vi "4Pi Objective Lock - EMBL_v2.vi"(7 "Calling VI Ref":refnum<vi>) -> ()   [LabVIEW 2021]
uses:
  <vilib>/Utility/miscctls.llb/LVPointTypeDef.ctl
  4Pi Objective Lock Type Defs/4Pi Obj Lock - Notifier Type.ctl
  4Pi Objective Lock Type Defs/4Pi Obj Lock - Actions.ctl
  <vilib>/vision/Image Controls.llb/IMAQ Image.ctl
  4Pi Objective Lock Type Defs/4Pi Obj Lock - Lock Settings.ctl
  Hardware Configuration/Hardware Configuration Controls/Device Type.ctl
  Hardware Configuration/Hardware Configuration Controls/Device Function.ctl
  4Pi Objective Lock Type Defs/4Pi Obj Lock - Camera Settings.ctl
  Device Library/Cameras/Camera Controls/Generic Camera ROI.ctl
  Device Library/Cameras/Camera Controls/Generic Camera Actions.ctl
  Device Manager/Common Device Queue/Common Device Controls/Common Device Actions.ctl
  Device Library/Stages/Stages Controls/Stage Actions.ctl
  <vilib>/addons/control/pid/pid.llb/PID (DBL Array).vi
  <vilib>/addons/control/pid/pid.llb/PID (DBL).vi
  <vilib>/addons/control/pid/NI_PID_pid.lvlib
  <vilib>/vision/NI_Vision_Development_Module.lvlib
panel:
  out "dz (µm)":dbl format="%.2f"
  out "dxy (px)":dbl[](array[numeric])
  in  "Main Tab":T1(tab)
  out "CC Max":cluster{"pixel size (µm)":dbl}(graph)
  out "Z Move":bool
  out "XY Move":bool
  out "Measured X Position (px)":dbl=1.0 format="%.3g"
  out "Measured Y Position (px)":dbl=1.0 format="%.3g"
  out "Measured sx/sy":dbl=1.0 format="%.3g"
  out "Target X Position (px)":dbl=1.0 format="%.3g"
  out "Target Y Position (px)":dbl=1.0 format="%.3g"
  out "Target sx/sy":dbl=1.0 format="%.3g"
  out "Z Axis Position (µm)":dbl=1.0 format="%.4g"
  out "Y Axis Position (µm)":dbl=1.0 format="%.2g"
  out "X Axis Position (µm)":dbl=1.0 format="%.2g"
  out "Z Target and Fit Value (µm)":T2(graph)
  in  "Start Lock":bool
  out "Y Target and Fit Position (µm)":T2(graph)
  out "X Target and Fit Position (µm)":T2(graph)
  in  "Restart Lock":bool
  out "Fit Error":bool
  out "Move Limit Error":bool
  out "dt z (s)":dbl format="%.3f"
  in  "Metric scale sx/sy":dbl=0.4
  in  "pixel size (µm)":dbl=0.05
  in  "X Update Scale Factor":dbl=0.005
  in  "Y Update Scale Factor":dbl=0.007
  in  "Z Update Scale Factor":dbl=0.4
  in  "Sample Z Step No.":u32=2
  in  "Sample Z Step Size (µm)":dbl=2.0
  in  "Update Delay (ms)":i32=10
  in  "D (Derivative)":dbl
  in  "I (Integral)":dbl
  in  "P (Proportional)":dbl=2.0
  in  "Invert Z Axis":bool
  in  "XY Drift Threshold":dbl=0.05
  in  "Abort If Error":bool
  in  "Flip XY Axis":bool
  in  "Invert X Axis":bool=TRUE
  in  "Invert Y Axis":bool=TRUE
  in  "Z Stage Move Limit (µm)":dbl=5.0
  in  "Z Drift Threshold":dbl=0.05
  in  "XY Stage Move Limit (µm)":dbl=1.0
  in  "Frame Accumulations":u16=10
  in  "XY Correction Active":bool=TRUE
  in  "Z Correction Active":bool=TRUE
  in  "Set Camera ROI":bool
  in  "Save Lock Settings":bool
  in  "Camera Settings":bool
  out "Target Y Position cc (px)":dbl=1.0 format="%.3g"
  out "Measured Y Position cc (px)":dbl=1.0 format="%.3g"
  out "Measured X Position cc (px)":dbl=1.0 format="%.3g"
  out "Target X Position cc (px)":dbl=1.0 format="%.3g"
  out "Target Z (µm)":dbl=1.0 format="%.3g"
  out "Measured Z (µm)":dbl=1.0 format="%.3g"
  out "CC Max Value":dbl=1.0 format="%.3g"
  in  "Quit":bool
  # "Z Drift Settings"
  # "XY Drift Settings"
  # "PID Control Values"
  # "General Settings"
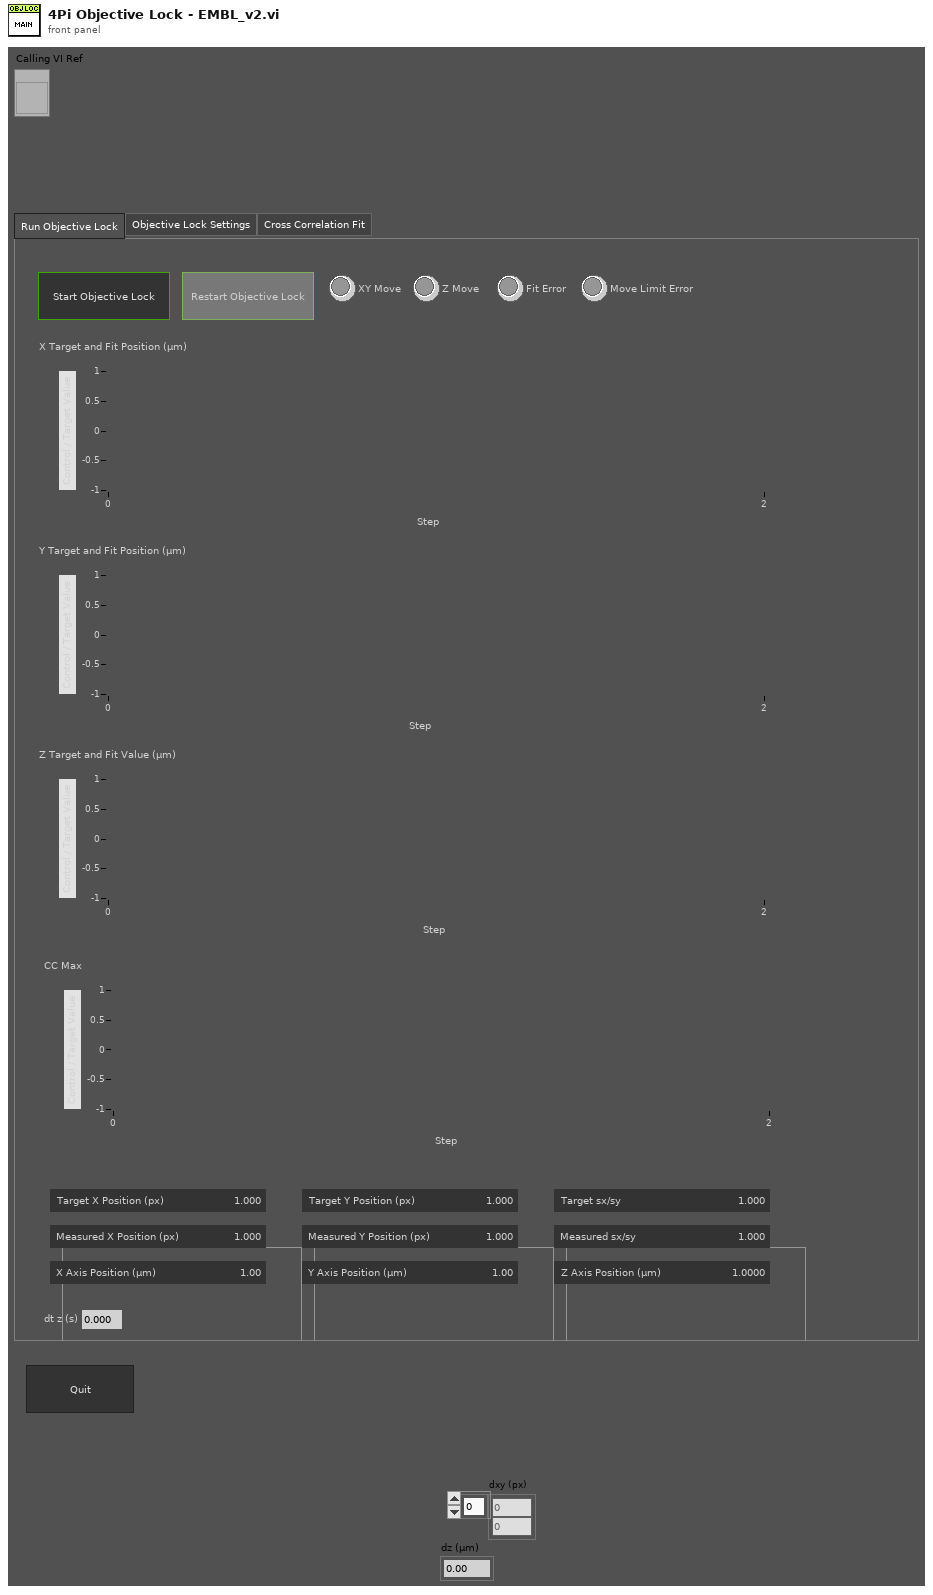
[diagram p1: front panel]
types:
  T1 = enum32{"Run Objective Lock", "Objective Lock Settings", "Cross Correlation Fit"}
  T2 = cluster{"Target 01":dbl, dbl, dbl, "Current 01":dbl, "Stage Pos":dbl, "Current 2":dbl}
  T3 = typedef "4Pi Obj Lock - Camera Settings.ctl" = cluster{"Exposure Time (s)":dbl, "H Offset":u16, "V Offset":u16, "H Width":u16, "V Width":u16}
  T4 = typedef "Device Function.ctl" = enum16{"Primary", "Secondary", "Overview", "Wide Field Drift Correction", "642 nm Excitation", "560 nm Excitation", "940 nm Excitation", "546 nm Excitation", "488 nm Excitation", "405 nm Excitation", "Objective Drift Correction", "4Pi Focus Lock", "4Pi Objective Lock", "Objective XY", "Objective Z", "Sample XY", "Sample Coarse Z", "Sample Z", "4Pi Lower", "4Pi Upper", "Em Small", "Em Large", "Ex Small", "Ex Large", "Mojo", "Adj Cavity", "Line Scanning", "Alert"}
  T5 = typedef "Device Type.ctl" = enum16{"AOTF", "Camera", "Deformable Mirror", "Laser", "Flip Mirror", "Shutter", "Stage", "Waveform", "FPGA", "Filter Wheel", "Email"}
  T6 = typedef "4Pi Obj Lock - Actions.ctl" = enum16{"Idle", "Start Lock", "Restart Lock", "Get Initial Position", "Get Target Z Position", "Get Ref Stack", "Cal Ref FFT", "Move To Init Z", "Get Current Image", "Get Current Z Position", "Get Current XY Position", "Get Current Position", "Check Drift", "Check Drift cc xy", "Check Drift cc z", "Check Drift cc", "Move XYZ", "Move XY", "Move Z", "Update Plots", "Delay", "Abort", "Exit Loop", "Quit"}
  T7 = typedef "4Pi Obj Lock - Lock Settings.ctl" = cluster{"Z Drift Threshold":dbl, "Z Stage Move Limit (µm)":dbl, "XY Drift Threshold":dbl, "XY Stage Move Limit (µm)":dbl, "Frame Accumulations":u16, "Abort If Error":bool, "Flip XY Axis":bool, "Invert X Axis":bool, "Invert Y Axis":bool, "Invert Z Axis":bool, "Z Correction Active":bool, "XY Correction Active":bool, "PID Values":dbl[], "Update Delay (ms)":i32, "Sample Z Step Size (µm)":dbl, "Sample Z Step No.":u32, "Z Update Scale Factor":dbl, "Y Update Scale Factor":dbl, "X Update Scale Factor":dbl}
  T8 = typedef "4Pi Obj Lock - Notifier Type.ctl" = cluster{"Actions":T6, "Z Drift Threshold":dbl, "Z Stage Move Limit (µm)":dbl, "XY Drift Threshold":dbl, "XY Stage Move Limit (µm)":dbl, "Frame Accumulations":u16, "Abort If Error":bool, "Z Correction Active":bool, "XY Correction Active":bool, "PID Values":dbl[], "Running?":bool, "Update Delay (ms)":i32, "Cur Image (SGL)":T9, "Ref Stack (SGL)":T9[], "Sample Z (µm)":dbl[], "Initial Z Position (µm)":dbl, "Z Step Size (µm)":dbl, "Z Step No.":u32, "Ref FFT Stack (CSG)":T9[], "CC Image (SGL) ":T9, "Tmp Image FFT (CSG)":T9[], "CC Image Max (SGL)":T9}
  T9 = typedef "IMAQ Image.ctl" = refnum<image>
  T10 = enum16{"Always On", "Always Off", "Off While Running"}
  T11 = typedef "LVPointTypeDef.ctl" = cluster{"Horizontal":i16, "Vertical":i16}
  T12 = typedef "Image Type" = u32
  T13 = typedef "Generic Camera Actions.ctl" = enum16{"Status", "Live Preview", "Capture", "Abort", "Set Exposure Time (s)", "Get Exposure Time (s)", "Set Gain", "Get Gain", "Set Gamma", "Get Gamma", "Record Settings", "Set ROI", "Get ROI", "Binning", "Defect Correction On/Off", "Cooler On/Off", "Fan On/Off", "Quit"}
  T14 = typedef "Generic Camera ROI.ctl" = cluster{"H_Offset":u16, "V_Offset":u16, "H_Width":u16, "V_Width":u16}
  T15 = typedef "Stage Actions.ctl" = enum16{"Get Position", "SERVO OFF", "SERVO ON", "SERVO ON/OFF", "MVR", "MOVE", "HALT", "ONTARGET", "ERROR", "REFERENCE", "INIT", "VELOCITY", "STATUS", "EXIT", "HOME", "ZEROPOS", "NANOPOS", "ANALOG", "QUIT"}
  T16 = enum32{"Invalid", "Standard", "Closed", "Hidden", "Minimized", "Maximized"}
  T17 = typedef "Common Device Actions.ctl" = enum16{"Specific Action", "Open Front Panel", "Close Front Panel", "Quit", "Quit All"}
  T18 = cluster{"Target 01":dbl, dbl, dbl, "Current 01":dbl, "Stage Pos":dbl, "Current 2":dbl}[]
  T19 = typedef "Stage Status.ctl" = enum16{"Error", "Abort", "Busy", "On Target"}
  T20 = typedef "2D Gaussian - Best Fit Parameters.ctl" = cluster{"Amplitude":dbl, "X Position":dbl, "Y Position":dbl, "X Width":dbl, "Y Width":dbl, "Offset":dbl}
  T21 = cluster{"PID Values[0]":dbl, "PID Values[1]":dbl, "PID Values[2]":dbl}
  T22 = cluster{"PID Values[0]":dbl, "PID Values[1]":dbl, "PID Values[2]":dbl}[]
  T23 = typedef "LVRectTypeDef.ctl" = cluster{"Left":i16, "Top":i16, "Right":i16, "Bottom":i16}
  T24 = typedef "LVBoundsTypeDef.ctl" = cluster{"Width":u32, "Height":u32}
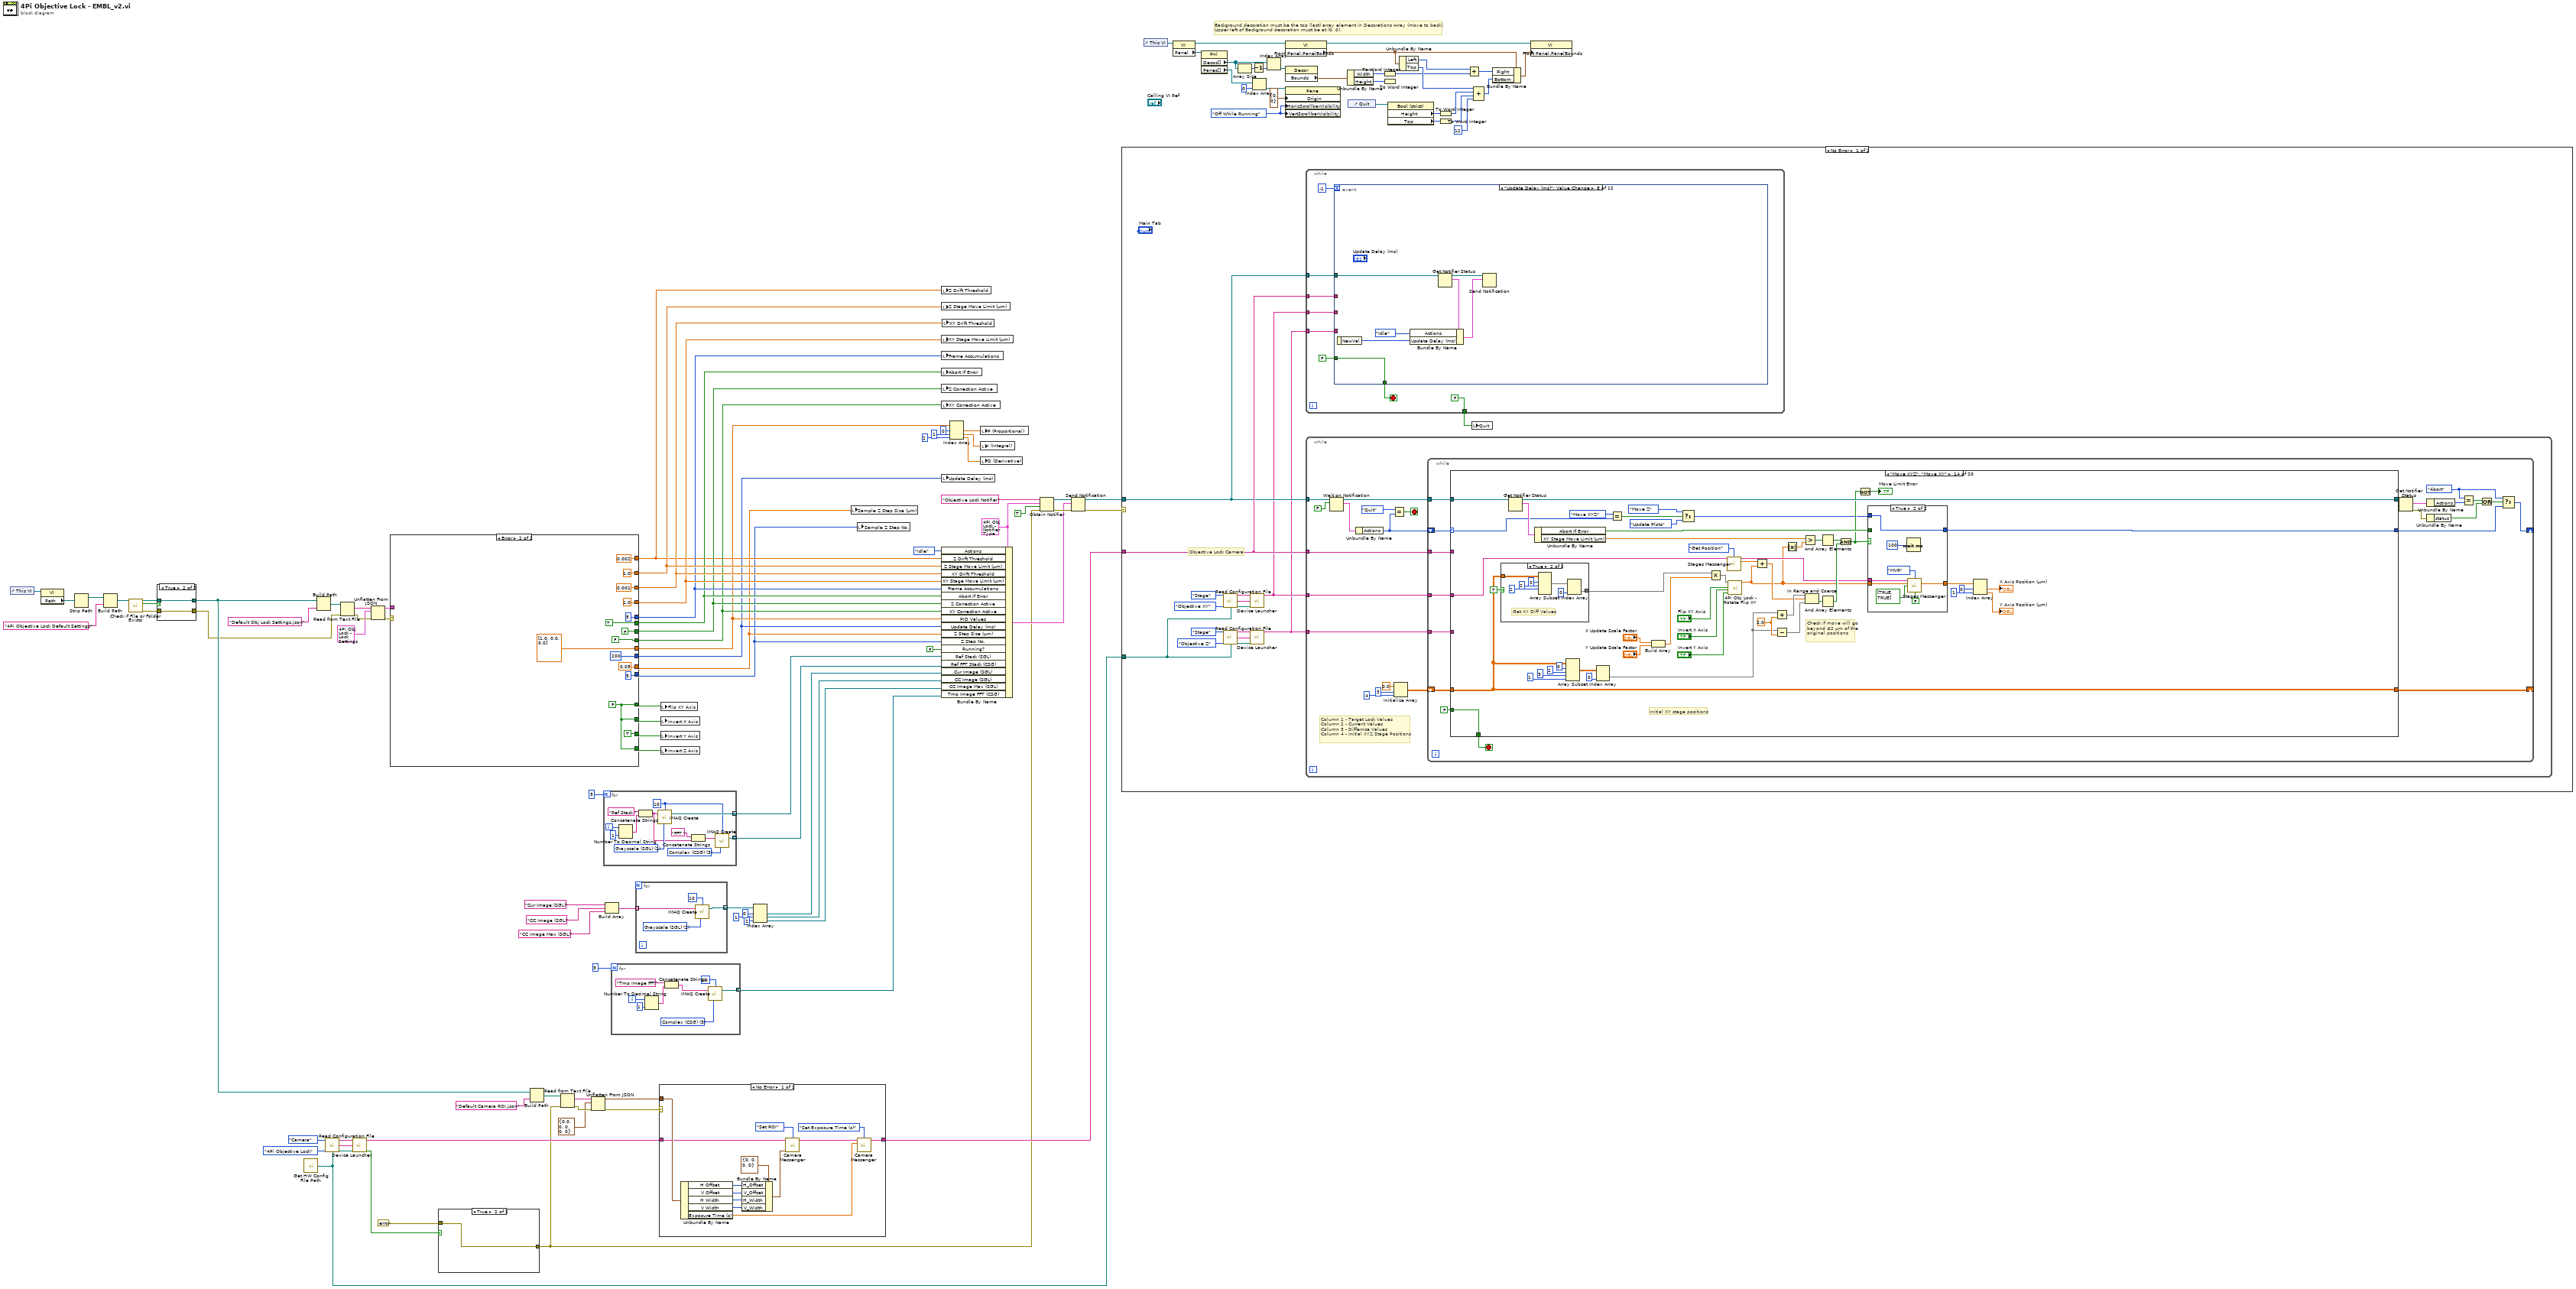
[diagram p0: block diagram]
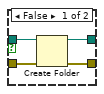
[diagram p2: hidden frame]
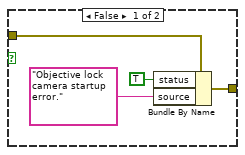
[diagram p3: hidden frame]
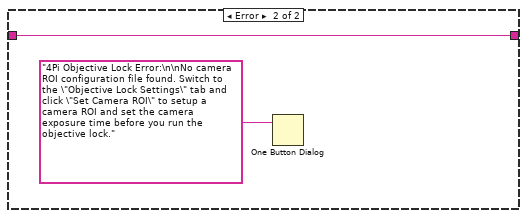
[diagram p4: hidden frame]
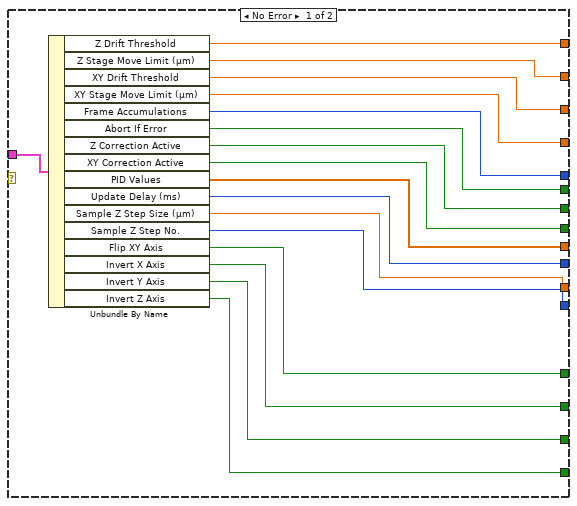
[diagram p5: hidden frame]
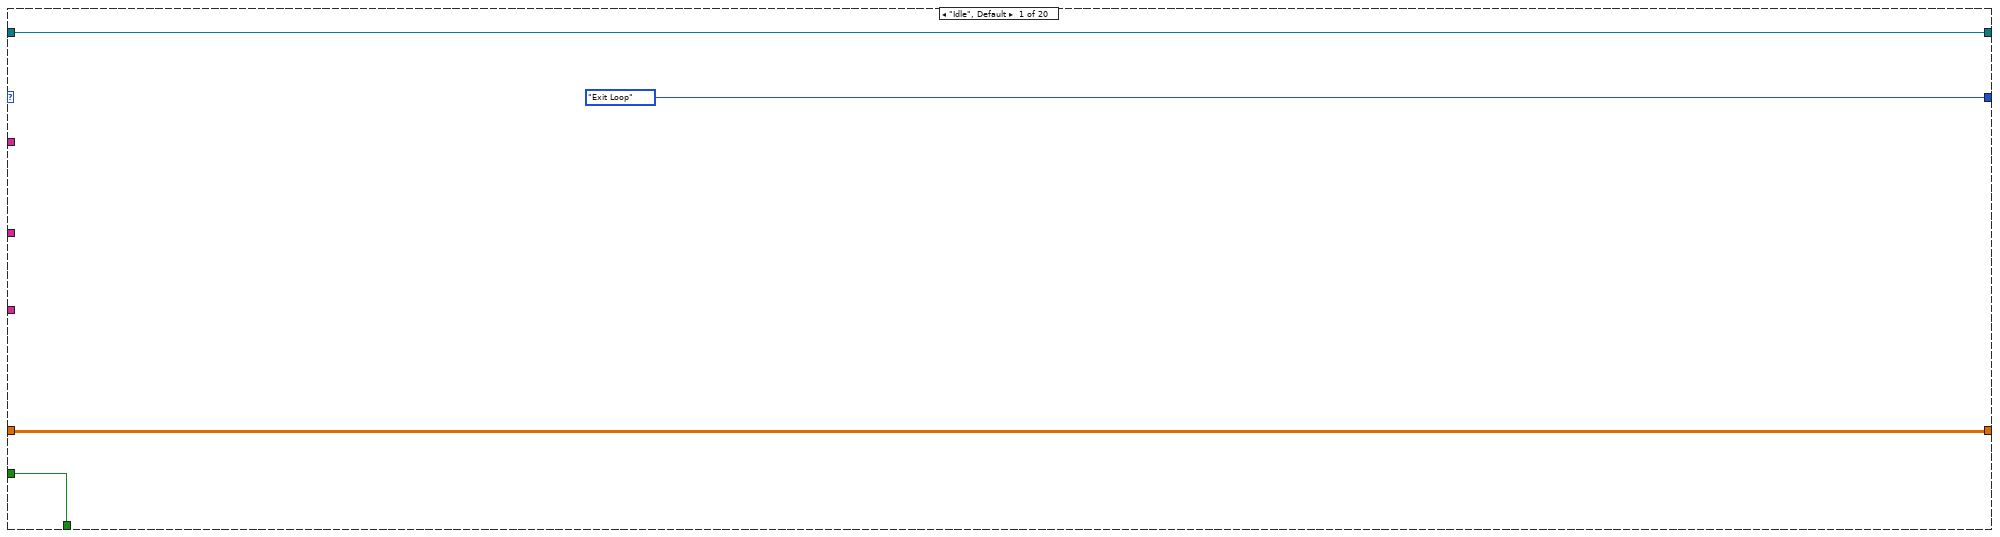
[diagram p6: hidden frame]
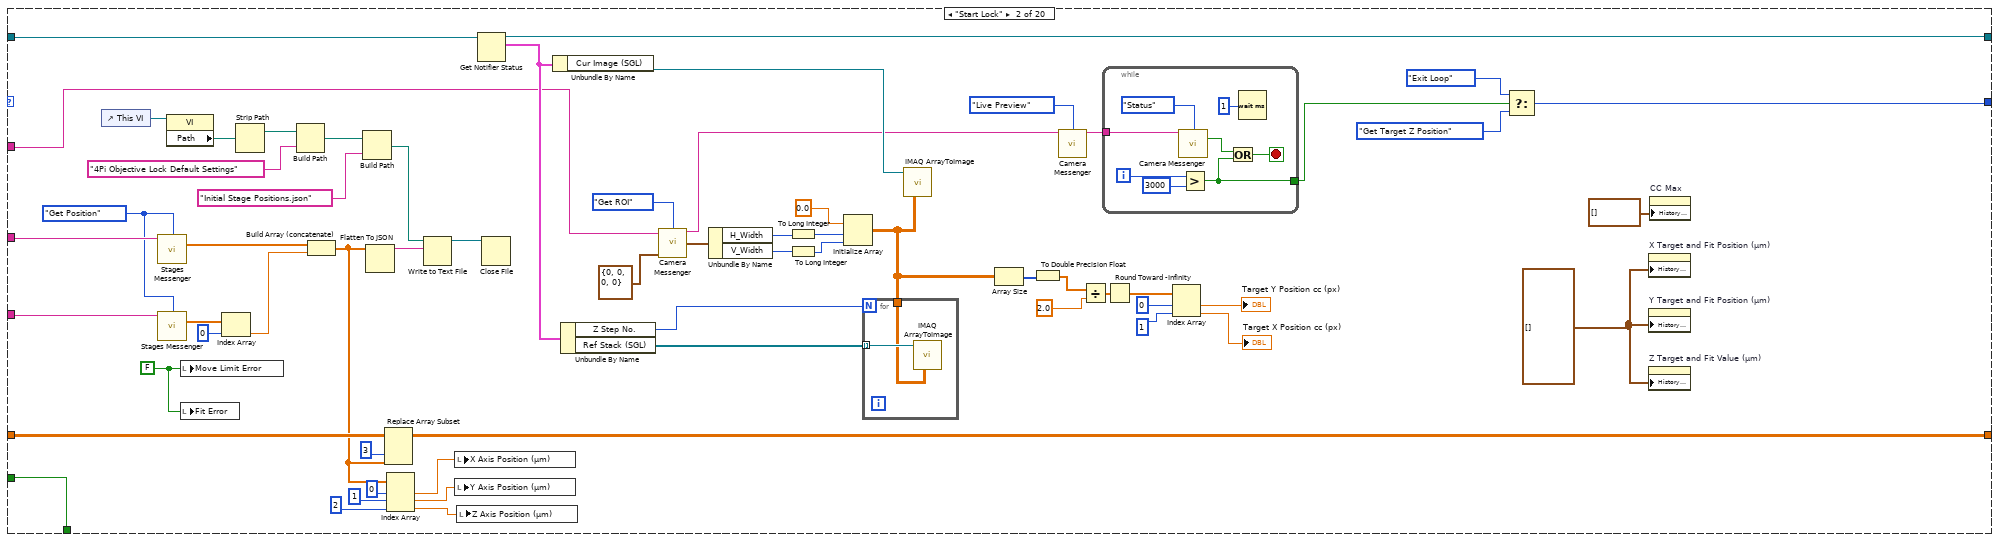
[diagram p7: hidden frame]
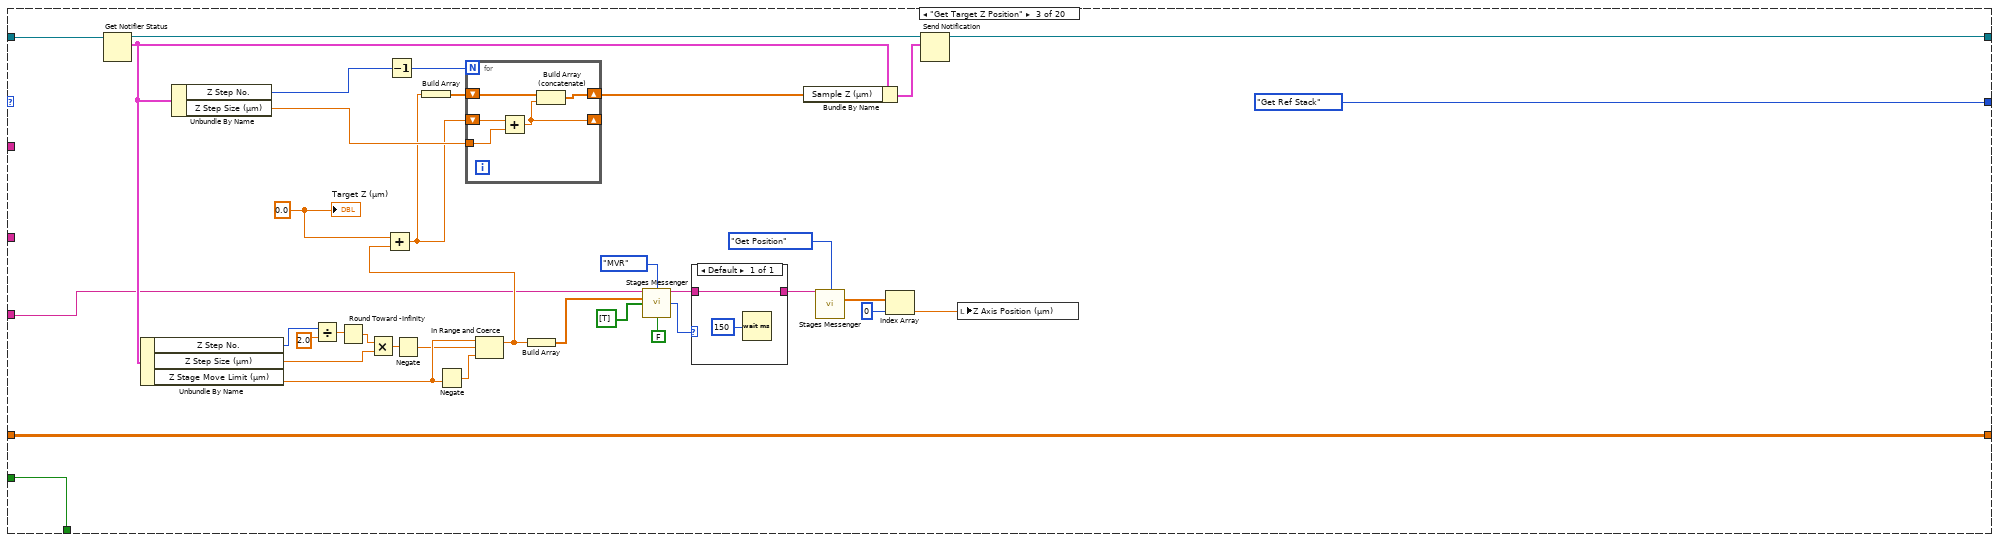
[diagram p8: hidden frame]
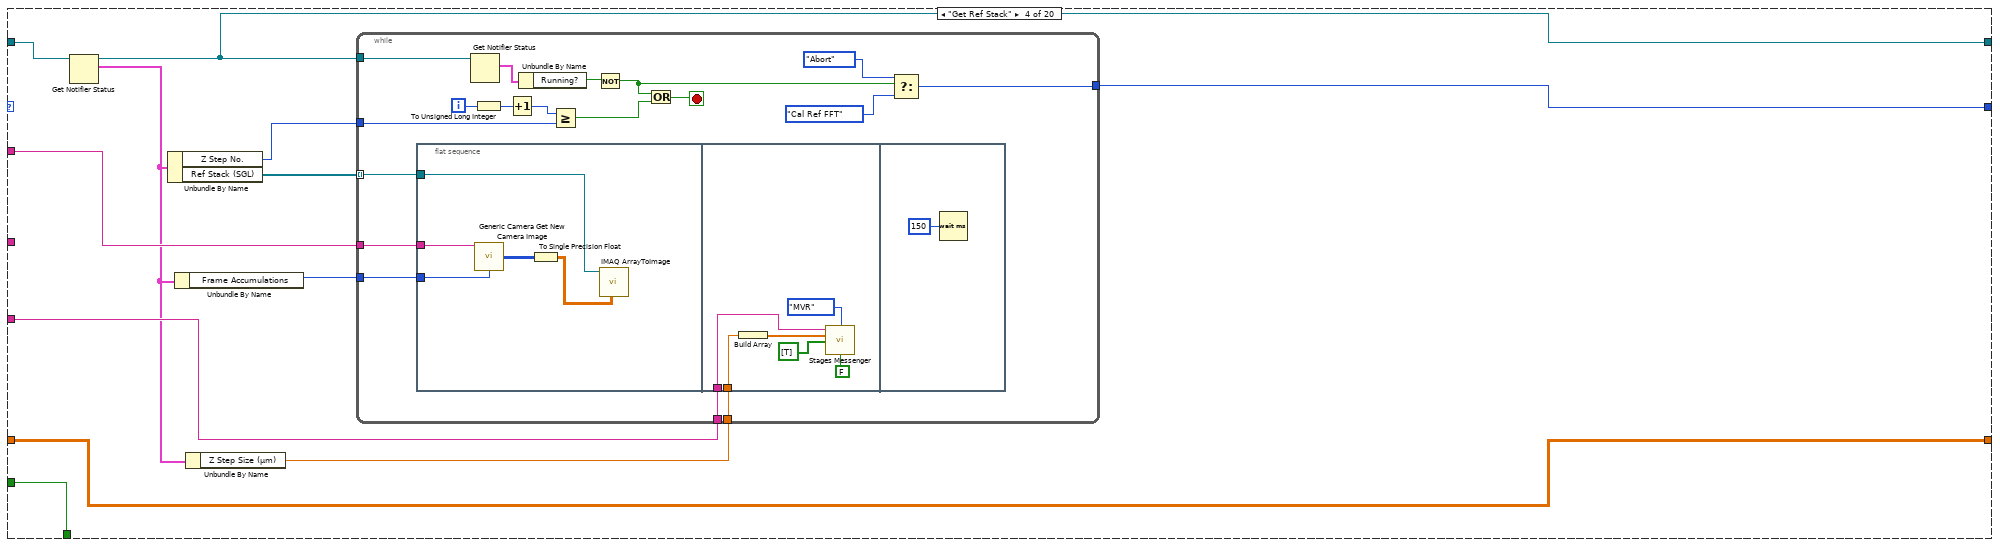
[diagram p9: hidden frame]
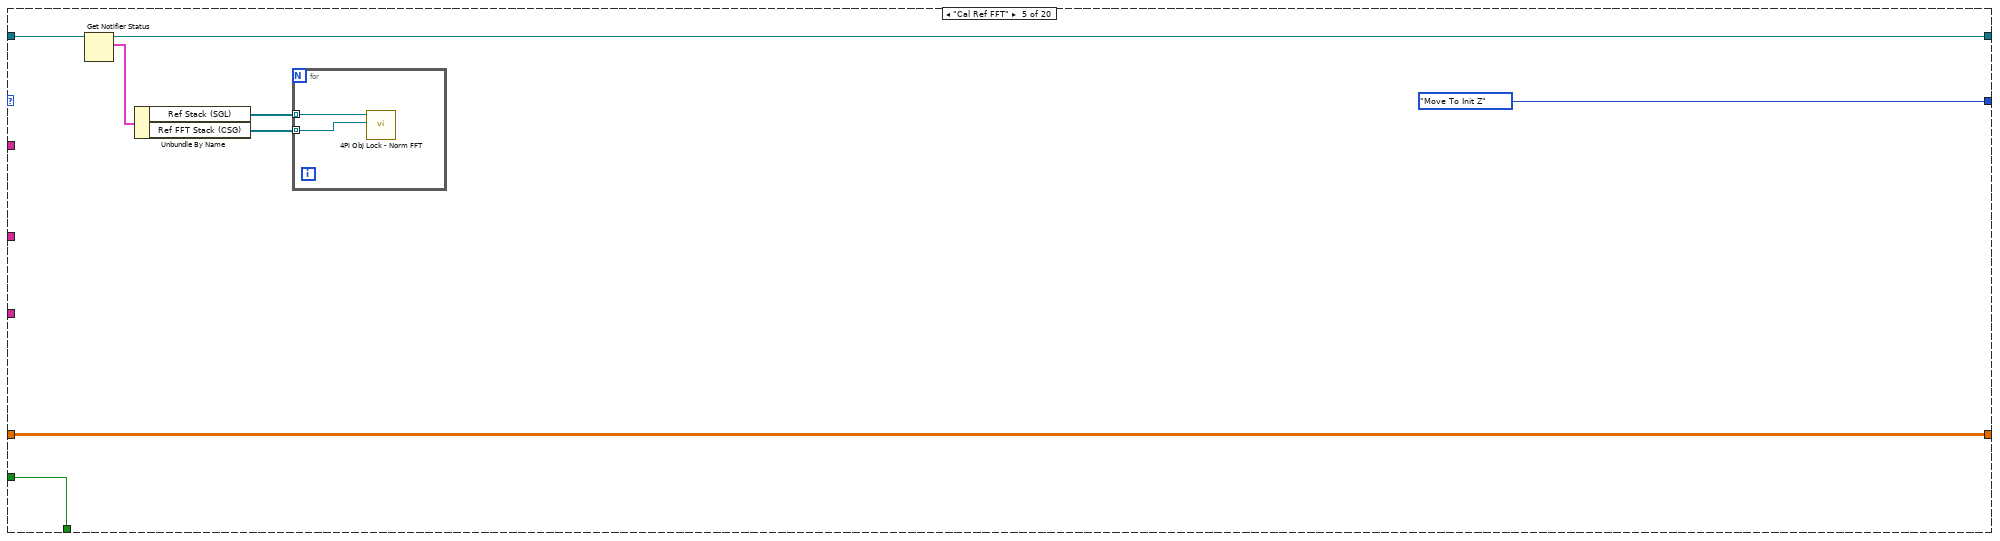
[diagram p10: hidden frame]
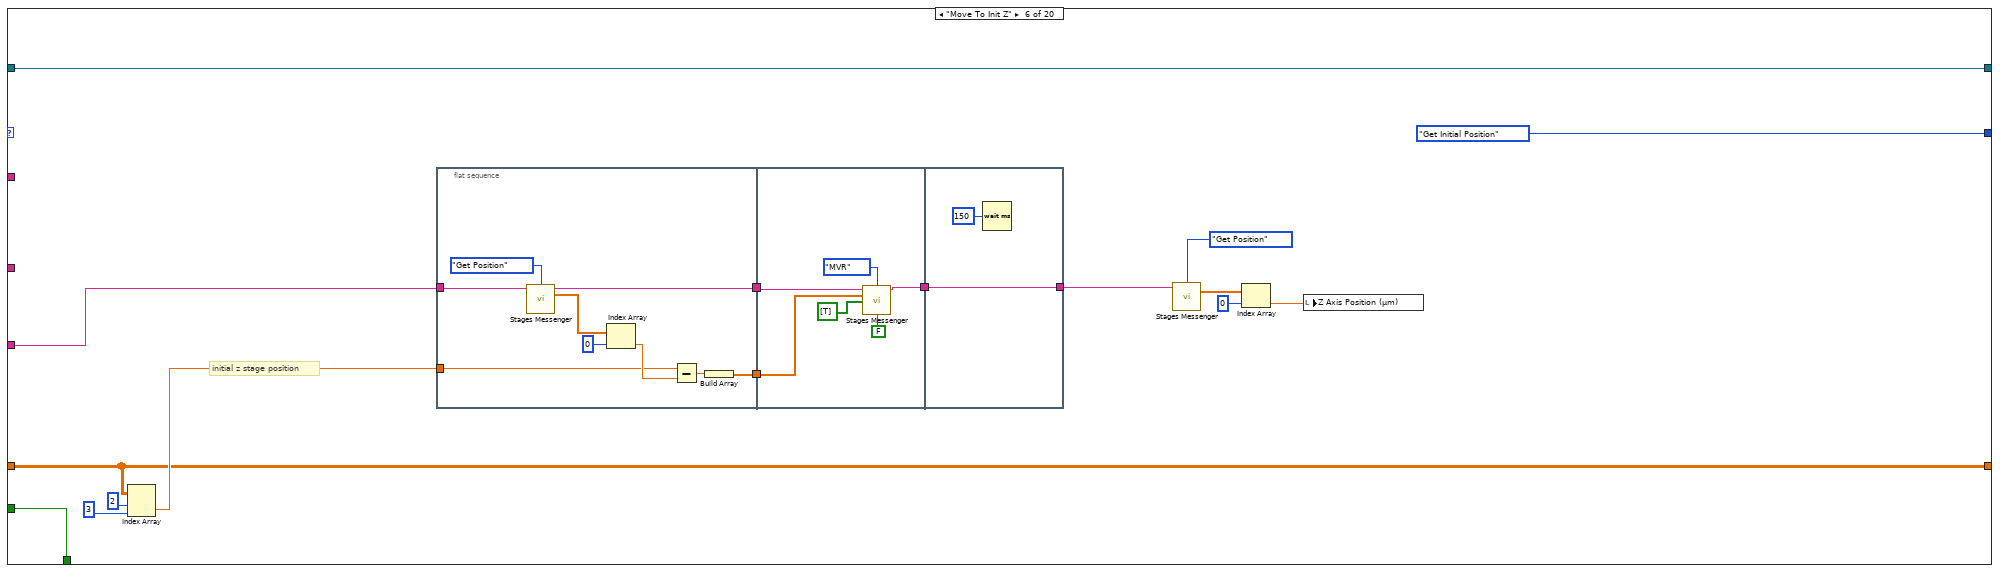
[diagram p11: hidden frame]
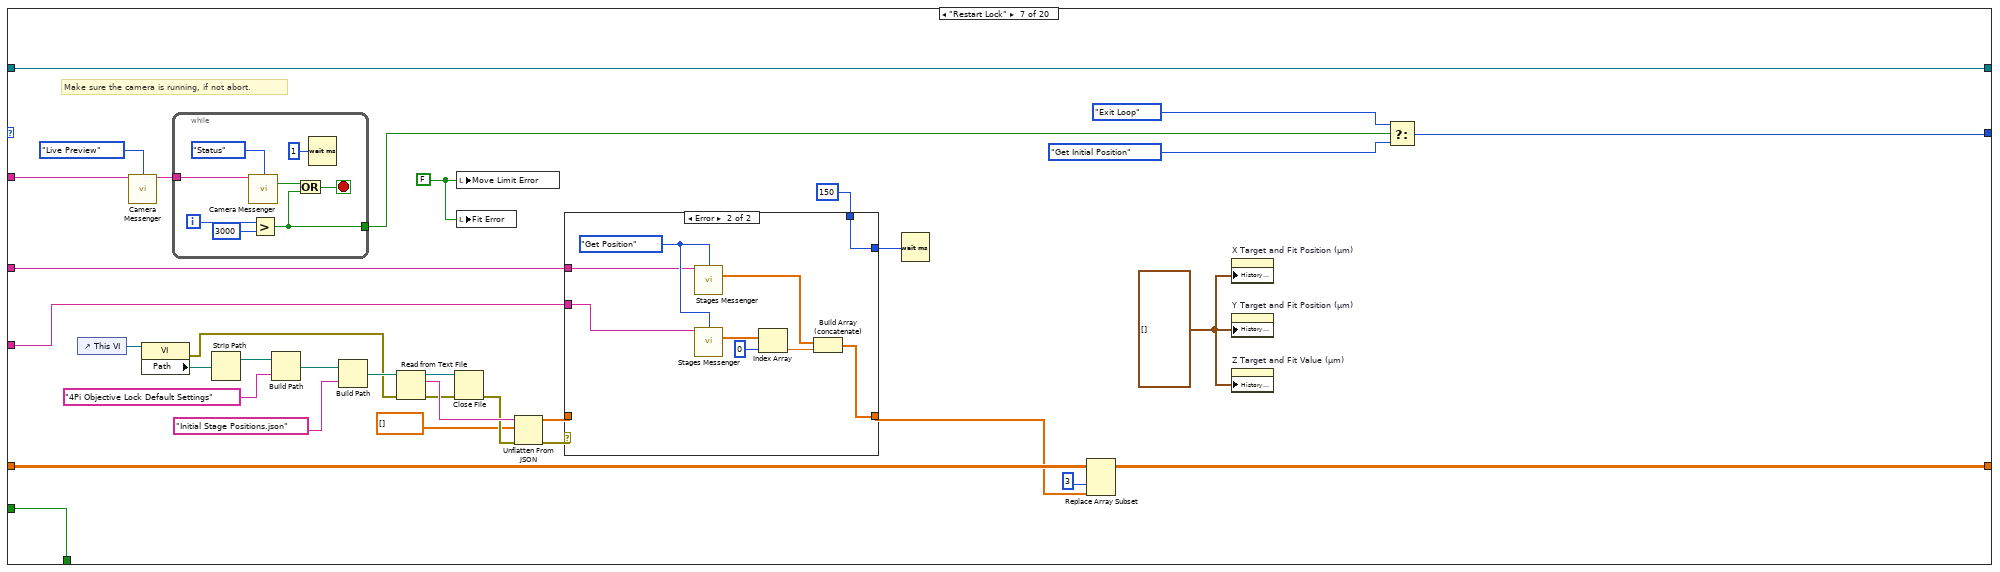
[diagram p12: hidden frame]
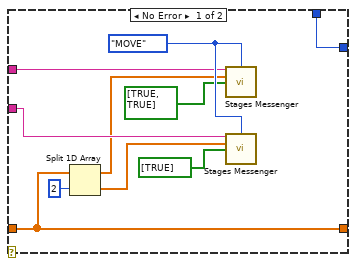
[diagram p13: hidden frame]
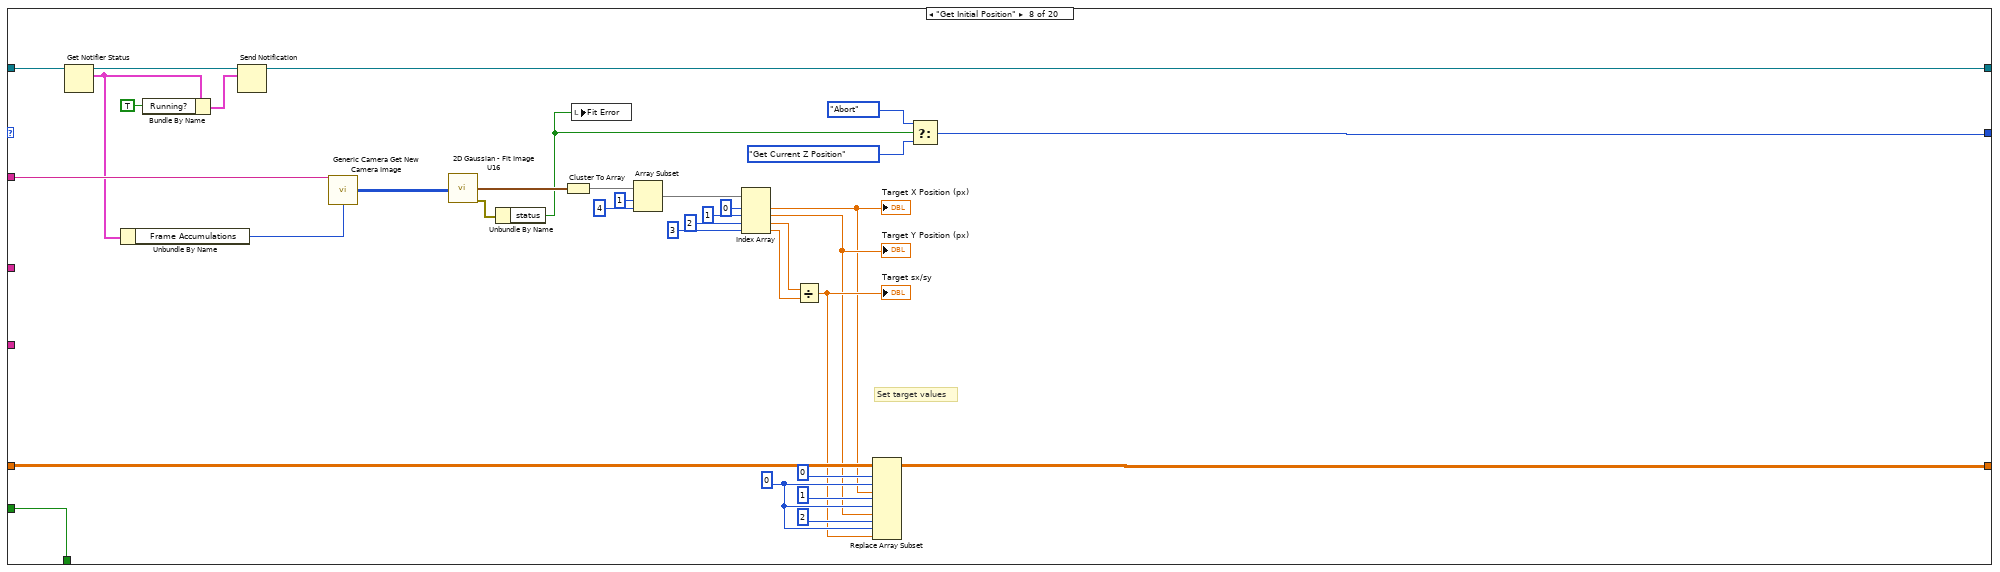
[diagram p14: hidden frame]
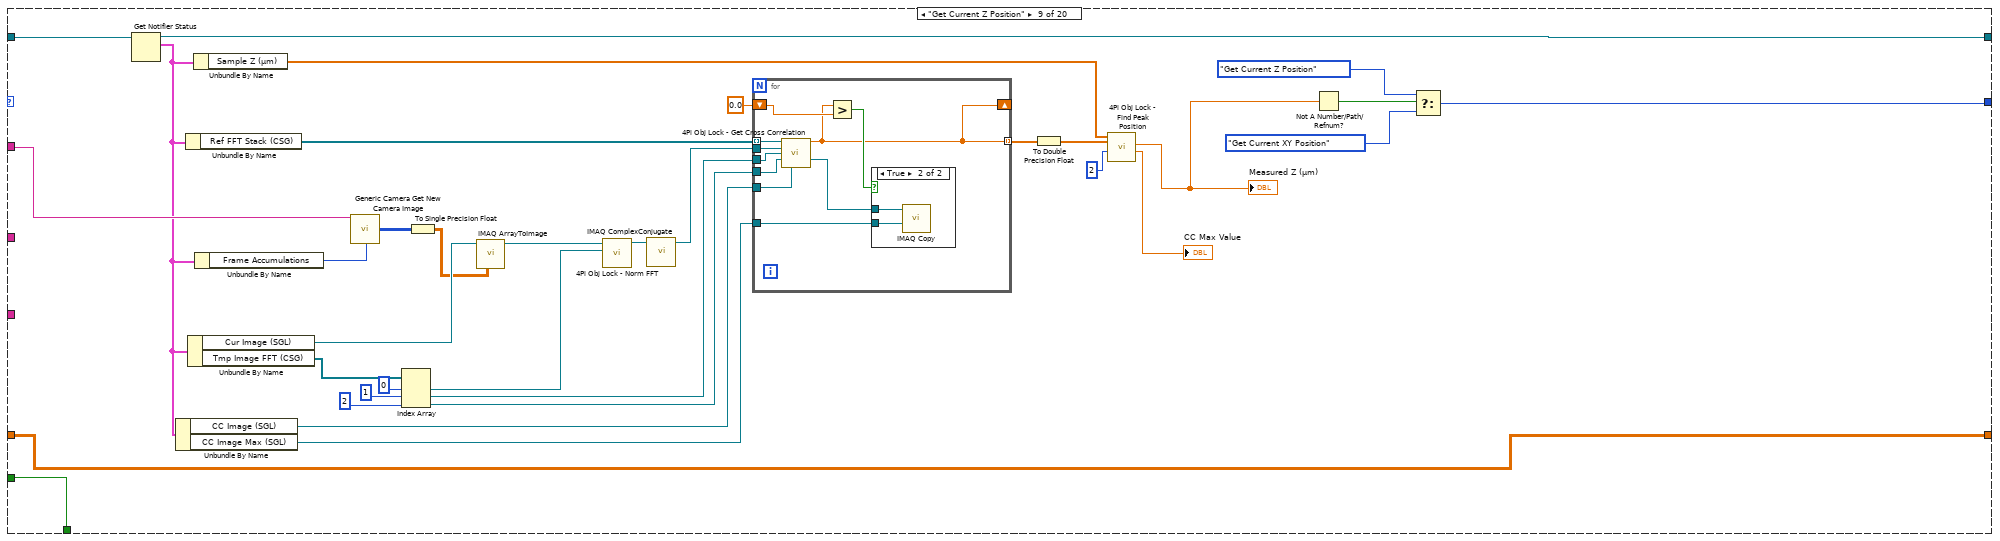
[diagram p15: hidden frame]
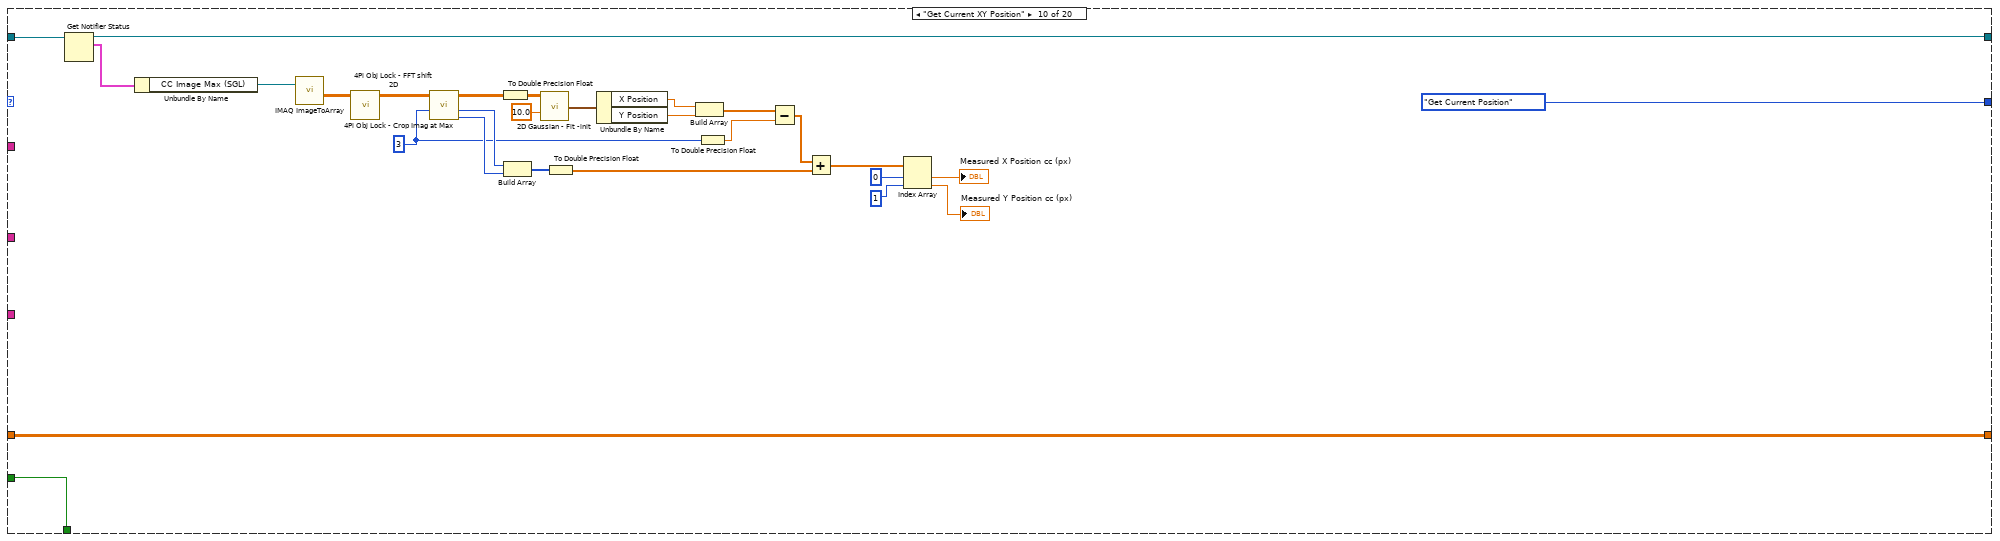
[diagram p17: hidden frame]
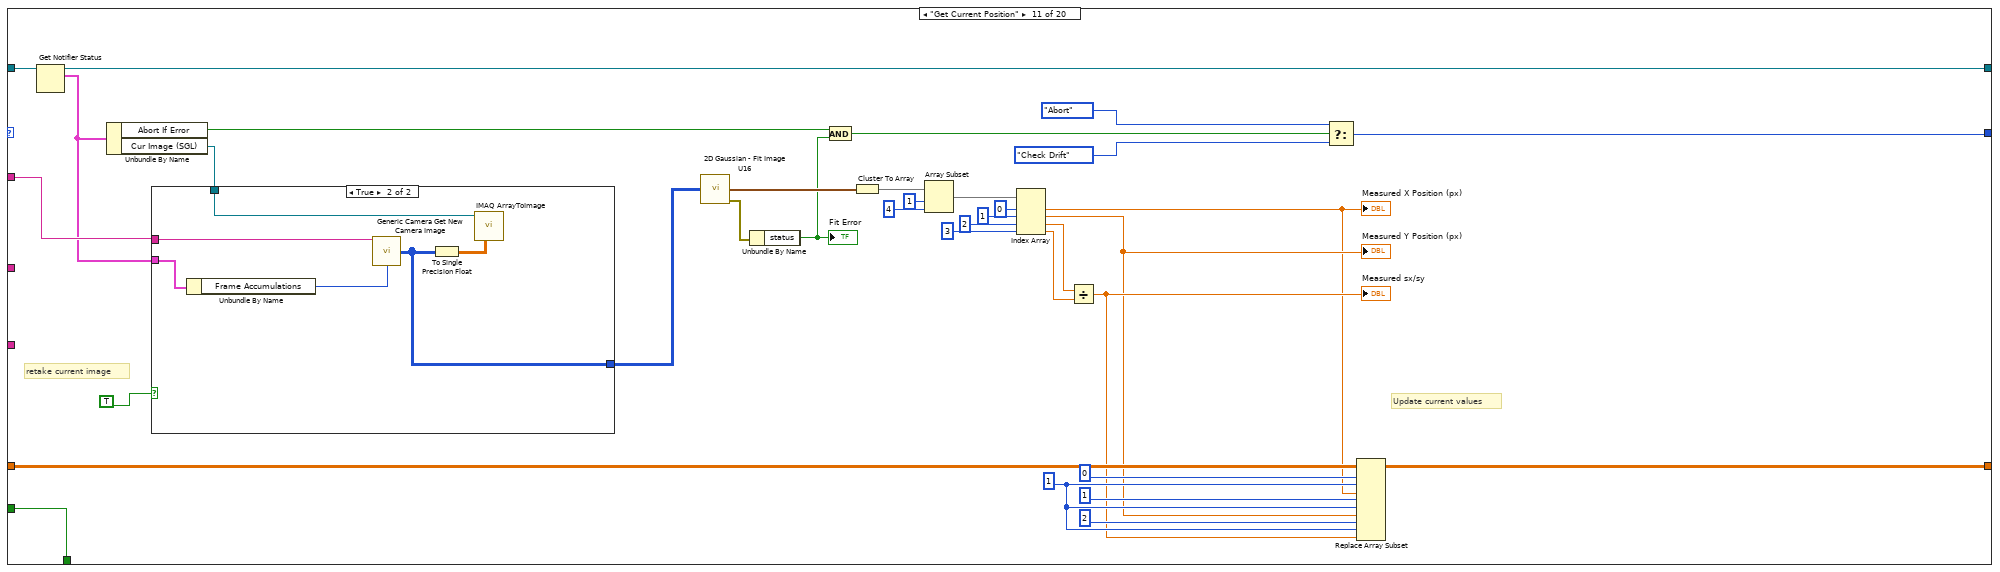
[diagram p18: hidden frame]
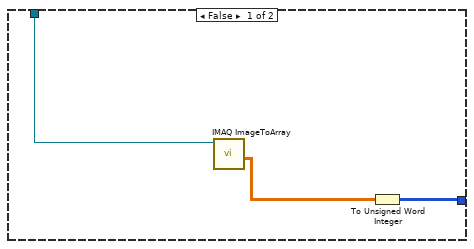
[diagram p19: hidden frame]
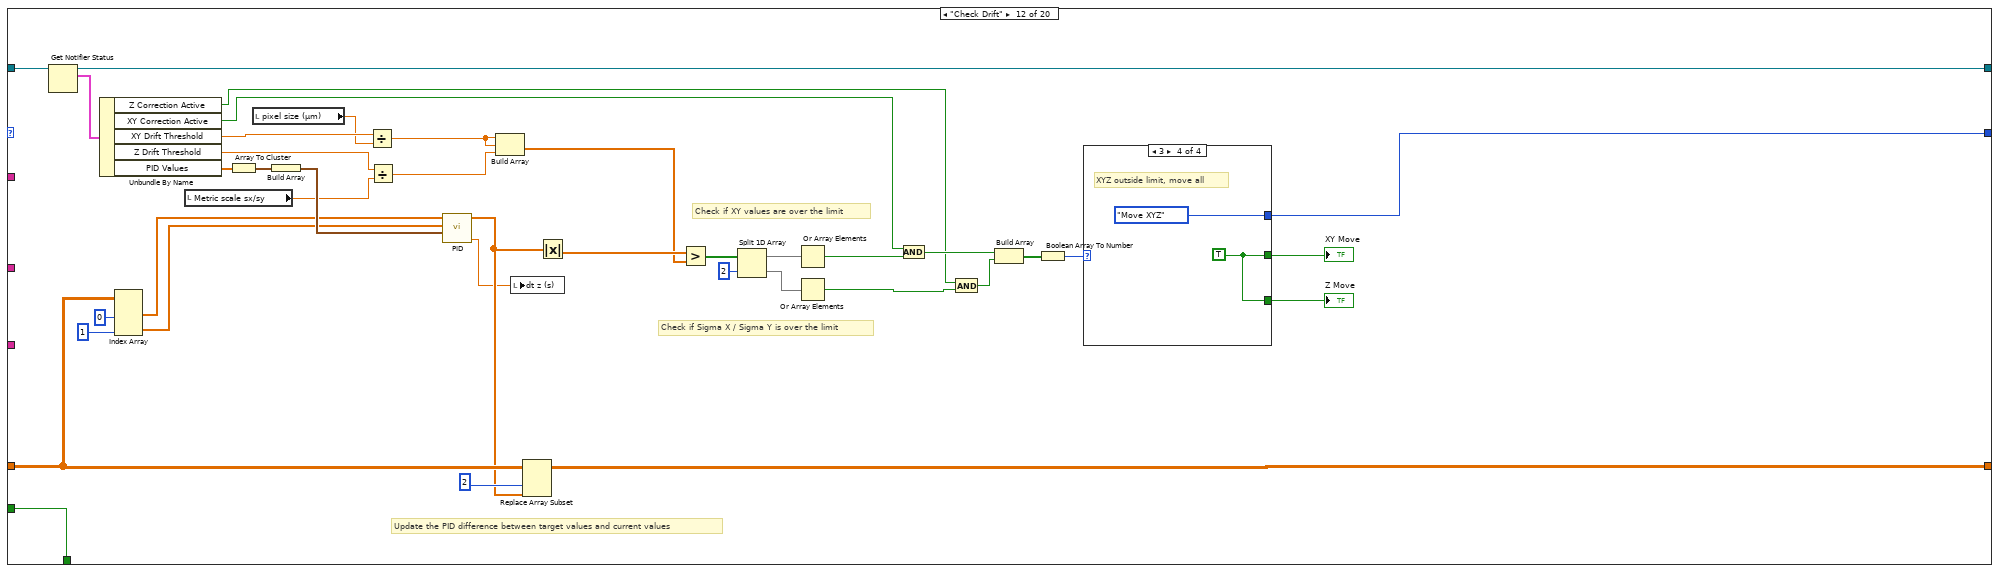
[diagram p20: hidden frame]
diagram:
  w78 = T8 {"Actions"=enum."Idle", "Z Drift Threshold"=0.05, "Z Stage Move Limit (µm)"=1.0, "XY Drift Threshold"=0.05, "XY Stage Move Limit (µm)"=1.0, "Frame Accumulations"=10, "Abort If Error"=FALSE, "Z Correction Active"=FALSE, "XY Correction Active"=FALSE, "PID Values"=[], "Running?"=FALSE, "Update Delay (ms)"=0, "Cur Image (SGL)"=refnum, "Ref Stack (SGL)"=[], "Sample Z (µm)"=[], "Initial Z Position (µm)"=0.0, "Z Step Size (µm)"=2.0, "Z Step No."=2, "Ref FFT Stack (CSG)"=[], "CC Image (SGL) "=refnum, "Tmp Image FFT (CSG)"=[], "CC Image Max (SGL)"=refnum} ("4Pi Obj Lock")
  w95 = T10."Off While Running" ("Vertical Scrollbar Visibility")
  # "Background decoration must be the top (last) array element in Decorations Array (move to back).\nUpper left of Background decoration must be at (0, 0)."
  n1 = control-ref of="This VI"() -> (w66:refnum<vi>)
  n2 = property class="VI"(reference=w66) -> ("Path"=w48:path)  [unwired: 1 in, 2 out]
  n3 = Strip Path(path=w48) -> (stripped path=w47:path)  [unwired: 1 out]
  n4 = Build Path(base path=w47, name or relative path="4Pi Objective Lock Default Settings") -> (appended path=w24:path)
  n5 = call <vilib>:"Check if File or Folder Exists.vi"("path"=w24) -> ("error out"=w20:errorcluster, "file or folder exists?"=w23:bool, "dup path"=w22:path)  [unwired: 8 in]
  n6 = case shown="True" w23 {
    tunnel: w22 -> [w116 w118]
    tunnel: [w115 w118] -> w21
    tunnel: w20 -> [w114 w117]
    tunnel: [w113 w117] -> w19
    frame False {
      n7 = Create Folder(path (use dialog)=w116, error in=w114) -> (created path=w115:path, error out=w113:errorcluster)  [unwired: 1 in, 1 out]
    }
    frame True {
    }
  }
  n8 = call "Get HW Config File Path.vi"() -> ("File Path"=w56:path)  [unwired: 14 in, 1 out]
  n9 = Build Path(base path=w21, name or relative path="Default Obj Lock Settings.json") -> (appended path=w75:path)
  n10 = call "Read Configuration File.vi"("Device Type"=Device_Type."Camera", "Device Function"=Device_Function."4Pi Objective Lock", "Config File Path"=w56) -> ("Unique Notifier Name"=w63:string, "Device Ports/IDs/Channels"=w65:string[], "Device Engine Path"=w64:path)  [unwired: 9 in, 1 out]
  n11 = Read from Text File(file (use dialog)=w75, error in=w19) -> (text=w74:string, error out=w73:errorcluster)  [unwired: 2 in, 2 out]
  n12 = call "Device Launcher.vi"("Notifier Name"=w63, "Device Ports/IDs/Channels"=w65, "Device Engine Path"=w64) -> ("Notifier Name"=w54:string, "Running?"=w60:bool)  [unwired: 11 in]
  n13 = Unflatten From JSON(JSON string=w74, type and defaults=T7 {"Z Drift Threshold"=0.05, "Z Stage Move Limit (µm)"=1.0, "XY Drift Threshold"=0.05, "XY Stage Move Limit (µm)"=1.0, "Frame Accumulations"=10, "Abort If Error"=FALSE, "Flip XY Axis"=FALSE, "Invert X Axis"=FALSE, "Invert Y Axis"=FALSE, "Invert Z Axis"=FALSE, "Z Correction Active"=TRUE, "XY Correction Active"=TRUE, "PID Values"=[], "Update Delay (ms)"=0, "Sample Z Step Size (µm)"=2.0, "Sample Z Step No."=2, "Z Update Scale Factor"=2.0, "Y Update Scale Factor"=2.0, "X Update Scale Factor"=2.0} ("Lock Settings"), error in (no error)=w73) -> (value=w70:T7, error out=w71:errorcluster)  [unwired: 4 in]
  n14 = case shown="Error" w71 {
    tunnel: [w134 0.002 ("Z Drift Threshold")] -> w25
    tunnel: [w133 1.0 ("Z Stage Move Limit (µm)")] -> w40
    tunnel: [w131 0.001 ("XY Drift Threshold")] -> w39
    tunnel: [w132 1.0 ("XY Stage Move Limit (µm)")] -> w38
    tunnel: [w130 u16 5 ("Frame Accumulations")] -> w37
    tunnel: [w129 TRUE ("Abort If Error")] -> w36
    tunnel: w70 -> [w135 _]
    tunnel: [w128 FALSE ("Z Correction Active")] -> w35
    tunnel: [w127 FALSE ("XY Correction Active")] -> w34
    tunnel: [w126 dbl[] [1.0, 0.0, 0.0] ("PID Values")] -> w33
    tunnel: [w125 u16 200 ("Update Delay (ms)")] -> w26
    tunnel: [w124 w139] -> w42
    tunnel: [w123 TRUE ("Invert Y Axis")] -> w43
    tunnel: [w122 w139] -> w44
    tunnel: [w121 w139] -> w45
    tunnel: [w120 0.05 ("Sample Z Step Size (µm)")] -> w5
    tunnel: [w119 u32 5 ("Sample Z Step No.")] -> w4
    frame No Error {
      n15 = Unbundle By Name(w135) -> ("Z Drift Threshold"=w134:dbl, "Z Stage Move Limit (µm)"=w133:dbl, "XY Drift Threshold"=w131:dbl, "XY Stage Move Limit (µm)"=w132:dbl, "Frame Accumulations"=w130:u16, "Abort If Error"=w129:bool, "Z Correction Active"=w128:bool, "XY Correction Active"=w127:bool, "PID Values"=w126:dbl[], "Update Delay (ms)"=w125:i32, "Sample Z Step Size (µm)"=w120:dbl, "Sample Z Step No."=w119:u32, "Flip XY Axis"=w121:bool, "Invert X Axis"=w122:bool, "Invert Y Axis"=w123:bool, "Invert Z Axis"=w124:bool)
    }
    frame Error {
      w139 = FALSE ("Flip XY Axis")
    }
  }
  n16 = case shown="True" w60 {
    tunnel: errorcluster {"status"=FALSE, "code"=0, "source"=""} ("Error") -> [w153 w154]
    tunnel: [w150 w154] -> w46
    frame False {
      n17 = Bundle By Name(cluster=w153, "status"=TRUE, "source"="Objective lock camera startup error." ("name or relative path")) -> (w150:errorcluster)
    }
    frame True {
    }
  }
  n18 = Build Path(base path=w21, name or relative path="Default Camera ROI.json") -> (appended path=w50:path)
  n19 = Read from Text File(file (use dialog)=w50, error in=w46) -> (text=w68:string, error out=w67:errorcluster)  [unwired: 2 in, 2 out]
  n20 = Unflatten From JSON(JSON string=w68, type and defaults=T3 {"Exposure Time (s)"=0.0, "H Offset"=0, "V Offset"=0, "H Width"=0, "V Width"=0} ("Camera Settings"), error in (no error)=w67) -> (value=w53:T3, error out=w58:errorcluster)  [unwired: 4 in]
  n21 = for {
    N: 5 -> [_]
    tunnel: [w166] -> w17 mode=indexing
    tunnel: [w155] -> w16 mode=indexing
    i -> [w165]
    w160 = T12 3 items=["Grayscale (U8)", "Grayscale (I16)", "Grayscale (SGL)", "Complex (CSG)", "RGB (U32)", "HSL (U32)", "RGB (U64)", "Grayscale (U16)"] ("Image Type")
    w161 = T12 2 items=["Grayscale (U8)", "Grayscale (I16)", "Grayscale (SGL)", "Complex (CSG)", "RGB (U32)", "HSL (U32)", "RGB (U64)", "Grayscale (U16)"] ("Image Type")
    w157 = 10 ("Border Size")
    n22 = Number To Decimal String(number=w165, width (-)=i16 1) -> (decimal integer string=w163:string)
    n23 = Concatenate Strings("Ref Stack " ("string"), w163) -> (w156:string)
    n24 = call "IMAQ Create"("Border Size"=w157, "Image Name"=w156, "Image Type"=w161) -> ("New Image"=w166:T9)  [unwired: 2 in, 1 out]
    n25 = Concatenate Strings("FFT " ("string"), w156) -> (w159:string)
    n26 = call "IMAQ Create"("Border Size"=w157, "Image Name"=w159, "Image Type"=w160) -> ("New Image"=w155:T9)  [unwired: 2 in, 1 out]
  }
  n27 = Build Array("Cur Image (SGL)" ("Image Name"), "CC Image (SGL)" ("Image Name"), "CC Image Max (SGL)" ("Image Name")) -> (w11:string[])
  n28 = for {
    N: 3 -> [_]
    tunnel: [w172] -> w6 mode=indexing
    i -> [w168]
    w173 = T12 3 items=["Grayscale (U8)", "Grayscale (I16)", "Grayscale (SGL)", "Complex (CSG)", "RGB (U32)", "HSL (U32)", "RGB (U64)", "Grayscale (U16)"] ("Image Type")
    n29 = Number To Decimal String(number=w168, width (-)=i16 1) -> (decimal integer string=w171:string)
    n30 = Concatenate Strings("Tmp Image FFT" ("Image Name"), w171) -> (w167:string)
    n31 = call "IMAQ Create"("Border Size"=10, "Image Name"=w167, "Image Type"=w173) -> ("New Image"=w172:T9)  [unwired: 2 in, 1 out]
  }
  n32 = for {
    tunnel: w11 -> [w176] mode=indexing
    tunnel: [w175] -> w10 mode=indexing
    w177 = T12 2 items=["Grayscale (U8)", "Grayscale (I16)", "Grayscale (SGL)", "Complex (CSG)", "RGB (U32)", "HSL (U32)", "RGB (U64)", "Grayscale (U16)"] ("Image Type")
    n33 = call "IMAQ Create"("Border Size"=10, "Image Name"=w176, "Image Type"=w177) -> ("New Image"=w175:T9)  [unwired: 2 in, 1 out]
  }
  n34 = case shown="No Error" w58 {
    tunnel: w54 -> [w182 w193]
    tunnel: w53 -> [w191 _]
    tunnel: [w179 w193] -> w52
    frame No Error {
      n35 = Unbundle By Name(w191) -> ("H Offset"=w186:u16, "V Offset"=w187:u16, "H Width"=w188:u16, "V Width"=w189:u16, "Exposure Time (s)"=w181:dbl)
      n36 = Bundle By Name(cluster=T14 {"H_Offset"=0, "V_Offset"=0, "H_Width"=0, "V_Width"=0} ("General Camera ROI"), "H_Offset"=w186, "V_Offset"=w187, "H_Width"=w188, "V_Width"=w189) -> (w185:T14)
      n37 = call "Camera Messenger.vi"("Notifier Name"=w182, "General Camera Actions"=Generic_Camera_Actions."Set ROI", "Camera ROI"=w185) -> ("Notifier Name Dup"=w180:string)  [unwired: 7 in, 5 out]
      n38 = call "Camera Messenger.vi"("Notifier Name"=w180, "General Camera Actions"=Generic_Camera_Actions."Set Exposure Time (s)", "Exposure Time (s)"=w181) -> ("Notifier Name Dup"=w179:string)  [unwired: 7 in, 5 out]
    }
    frame Error {
      n39 = One Button Dialog(message="4Pi Objective Lock Error:\n\nNo camera ROI configuration file found. Switch to the \"Objective Lock Settings\" tab and click \"Set Camera ROI\" to setup a camera ROI and set the camera exposure time before you run the objective lock.") -> ()  [unwired: 1 in, 1 out]
    }
  }
  n40 = local write "Flip XY Axis"(w45) -> ()
  n41 = local write "Invert X Axis"(w44) -> ()
  n42 = local write "Invert Y Axis"(w43) -> ()
  n43 = local write "Invert Z Axis"(w42) -> ()
  n44 = Index Array(array=w10, index #1=0 ("index"), index #2=1 ("index"), index #3=2 ("index")) -> (element #1=w9:T9, element #2=w8:T9, element #3=w1:T9)
  n45 = local write "Sample Z Step Size (µm)"(w5) -> ()
  n46 = local write "Sample Z Step No."(w4) -> ()
  n47 = Bundle By Name(cluster=w78, "Actions"=4Pi_Obj_Lock_-_Actions."Idle", "Z Drift Threshold"=w25, "Z Stage Move Limit (µm)"=w40, "XY Drift Threshold"=w39, "XY Stage Move Limit (µm)"=w38, "Frame Accumulations"=w37, "Abort If Error"=w36, "Z Correction Active"=w35, "XY Correction Active"=w34, "PID Values"=w33, "Update Delay (ms)"=w26, "Z Step Size (µm)"=w5, "Z Step No."=w4, "Running?"=FALSE ("Obj Lock Active?"), "Ref Stack (SGL)"=w17, "Ref FFT Stack (CSG)"=w16, "Cur Image (SGL)"=w9, "CC Image (SGL)"=w8, "CC Image Max (SGL)"=w1, "Tmp Image FFT (CSG)"=w6) -> (w77:T8)
  n48 = local write "Z Drift Threshold"(w25) -> ()
  n49 = local write "Z Stage Move Limit (µm)"(w40) -> ()
  n50 = local write "XY Stage Move Limit (µm)"(w38) -> ()
  n51 = local write "Frame Accumulations"(w37) -> ()
  n52 = local write "Abort If Error"(w36) -> ()
  n53 = local write "Z Correction Active"(w35) -> ()
  n54 = local write "XY Correction Active"(w34) -> ()
  n55 = local write "Update Delay (ms)"(w26) -> ()
  n56 = local write "XY Drift Threshold"(w39) -> ()
  n57 = Index Array(array=w33, index #1=0 ("index"), index #2=1 ("index"), index #3=2 ("index")) -> (element #1=w29:dbl, element #2=w27:dbl, element #3=w28:dbl)
  n58 = local write "P (Proportional)"(w29) -> ()
  n59 = local write "I (Integral)"(w27) -> ()
  n60 = local write "D (Derivative)"(w28) -> ()
  n61 = Obtain Notifier(name (unnamed)="Objective Lock Notifier", notification data type=w78, create if not found? (T)=TRUE, error in (no error)=w46) -> (notifier out=w80:refnum<notifier>, error out=w81:errorcluster)  [unwired: 1 out]
  n62 = Send Notification(notification=w77, notifier=w80, error in (no error)=w81) -> (notifier out=w79:refnum<notifier>, error out=w57:errorcluster)
  n63 = case shown="No Error" w57 {
    tunnel: w56 -> [w198 _]
    tunnel: w79 -> [w196 _]
    tunnel: w52 -> [w197 _]
    frame No Error {
      # "Objective Lock Camera"
      n64 = call "Read Configuration File.vi"("Device Type"=Device_Type."Stage", "Device Function"=Device_Function."Objective XY", "Config File Path"=w198) -> ("Unique Notifier Name"=w206:string, "Device Ports/IDs/Channels"=w204:string[], "Device Engine Path"=w205:path)  [unwired: 9 in, 1 out]
      n65 = call "Read Configuration File.vi"("Device Type"=Device_Type."Stage", "Device Function"=Device_Function."Objective Z", "Config File Path"=w198) -> ("Unique Notifier Name"=w201:string, "Device Ports/IDs/Channels"=w203:string[], "Device Engine Path"=w202:path)  [unwired: 9 in, 1 out]
      n66 = call "Device Launcher.vi"("Notifier Name"=w206, "Device Ports/IDs/Channels"=w204, "Device Engine Path"=w205) -> ("Notifier Name"=w195:string)  [unwired: 11 in, 1 out]
      n67 = call "Device Launcher.vi"("Notifier Name"=w201, "Device Ports/IDs/Channels"=w203, "Device Engine Path"=w202) -> ("Notifier Name"=w194:string)  [unwired: 11 in, 1 out]
      n68 = while {
        tunnel: [FALSE] -> w209
        tunnel: w197 -> [w1067]
        tunnel: w196 -> [w1066]
        tunnel: w195 -> [w1065]
        tunnel: w194 -> [w1064]
        stop <- w1069 stop-if-true
        n69 = event shown="[7] \"Update Delay (ms)\": Value Change" {
          selector: _ -> [_ _ _ _ _ _ _ _ _ _ _ _]
          dyn-events: _ -> [_ _ _ _ _ _ _ _ _ _ _ _]
          timeout: -1 -> [_ _ _ _ _ _ _ _ _ _ _ _]
          tunnel: FALSE -> [w1072 w1076 w1081 w1097 w1117 w1152 w1179 w1186 w1215 w1225 w1232 _]
          tunnel: [w1072 w1076 w1081 w1097 w1117 w1152 w1179 w1186 w1215 w1225 w1232 w1242] -> w1069
          tunnel: w1067 -> [_ _ w1080 _ _ _ _ _ _ _ _ _]
          tunnel: w1066 -> [_ _ _ w1096 w1114 w1155 w1178 w1185 w1214 w1224 w1231 w1237]
          tunnel: w1065 -> [_ _ _ _ _ _ _ _ _ _ _ _]
          tunnel: w1064 -> [_ _ _ _ _ _ _ _ _ _ _ _]
          event Timeout {
            n70 = event-data() -> ()  [unwired: 1 in, 1 out]
          }
          event Application Instance Close? {
            n71 = event-data() -> ()  [unwired: 1 in, 1 out]
            n72 = control-ref of="This VI"() -> (w1073:refnum<vi>)
            n73 = invoke class="VI" method="FP.Open"(reference=w1073, "Activate"=TRUE ("Activate?"), "State"=T16."Standard") -> ()  [unwired: 2 in, 5 out]
            n74 = event-data("Discard?"=TRUE) -> ()  [unwired: 1 in, 1 out]
          }
          event "Set Camera ROI", "Camera Settings": Value Change {
            n75 = event-data() -> ("CtlRef"=w1079:refnum<vi>)  [unwired: 1 in]
            n76 = property class="Bool"(reference=w1079) -> ("Label.Text"=w1078:string)  [unwired: 1 in, 2 out]
            n77 = case shown="\"Camera Settings\"" w1078 {
              tunnel: w1080 -> [_ w1083 w1087]
              frame Default {
              }
              frame "Camera Settings" {
                n78 = Select(t=Common_Device_Actions."Open Front Panel" ("Common Action"), s="Camera Settings", f=Common_Device_Actions."Close Front Panel") -> (s? t:f=w1084:T17)
                n79 = call "Common Device Queue Messenger.vi"("Common Action"=w1084, "Notifier Name"=w1083) -> ()  [unwired: 13 in, 1 out]
              }
              frame "Set Camera ROI" {
                n80 = call "4Pi Obj Lock - Setup Camera.vi"("Camera Notifier Name"=w1087) -> ()  [unwired: 14 in, 1 out]
              }
            }
          }
          event "XY Correction Active", "Z Correction Active", "Abort If Error": Value Change {
            n81 = event-data() -> ("NewVal"=w1092:bool, "CtlRef"=w1095:refnum<vi>)  [unwired: 1 in]
            n82 = Get Notifier Status(notifier=w1096) -> (notifier out=w1094:refnum<notifier>, current notification=w1091:T8)  [unwired: 1 in, 3 out]
            n83 = property class="Bool (strict)"(reference=w1095) -> ("Label.Text"=w1093:string)  [unwired: 1 in, 2 out]
            n84 = case shown="\"XY Correction Active\"" w1093 {
              tunnel: w1092 -> [_ w1100 w1103 w1106]
              tunnel: w1091 -> [w1098 w1101 w1104 w1107]
              tunnel: [w1098 w1099 w1102 w1105] -> w1090
              frame Default {
              }
              frame "XY Correction Active" {
                n85 = Bundle By Name(cluster=w1101, "XY Correction Active"=w1100) -> (w1099:T8)
              }
              frame "Z Correction Active" {
                n86 = Bundle By Name(cluster=w1104, "Z Correction Active"=w1103) -> (w1102:T8)
              }
              frame "Abort If Error" {
                n87 = Bundle By Name(cluster=w1107, "Abort If Error"=w1106) -> (w1105:T8)
              }
            }
            n88 = Bundle By Name(cluster=w1090, "Actions"=4Pi_Obj_Lock_-_Actions."Idle") -> (w1088:T8)
            n89 = Send Notification(notification=w1088, notifier=w1094) -> ()  [unwired: 1 in, 2 out]
          }
          event "Z Drift Threshold", "Z Stage Move Limit (µm)", "XY Drift Threshold", "XY Stage Move Limit (µm)", "P (Proportional)", "I (Integral)", "D (Derivative)", "Sample Z Step Size (µm)": Value Change {
            n90 = event-data() -> ("NewVal"=w1112:dbl, "CtlRef"=w1113:refnum<vi>)  [unwired: 1 in]
            n91 = Get Notifier Status(notifier=w1114) -> (notifier out=w1111:refnum<notifier>, current notification=w1115:T8)  [unwired: 1 in, 3 out]
            n92 = property class="DigNum (strict)"(reference=w1113) -> ("Label.Text"=w1116:string)  [unwired: 1 in, 2 out]
            n93 = case shown="\"Sample Z Step Size (µm)\"" w1116 {
              tunnel: w1112 -> [_ w1120 w1123 w1126 w1129 w1134 w1140 w1146 w1150]
              tunnel: w1115 -> [w1118 w1121 w1124 w1127 w1130 w1133 w1139 w1145 w1151]
              tunnel: [w1118 w1119 w1122 w1125 w1128 w1131 w1137 w1143 w1149] -> w1109
              frame Default {
              }
              frame "Z Drift Threshold" {
                n94 = Bundle By Name(cluster=w1121, "Z Drift Threshold"=w1120) -> (w1119:T8)
              }
              frame "Z Stage Move Limit (µm)" {
                n95 = Bundle By Name(cluster=w1124, "Z Stage Move Limit (µm)"=w1123) -> (w1122:T8)
              }
              frame "XY Drift Threshold" {
                n96 = Bundle By Name(cluster=w1127, "XY Drift Threshold"=w1126) -> (w1125:T8)
              }
              frame "XY Stage Move Limit (µm)" {
                n97 = Bundle By Name(cluster=w1130, "XY Stage Move Limit (µm)"=w1129) -> (w1128:T8)
              }
              frame "P (Proportional)" {
                n98 = Unbundle By Name(w1133) -> ("PID Values"=w1136:dbl[])
                n99 = Replace Array Subset(array=w1136, new element=w1134, index=0) -> (w1132:dbl[])
                n100 = Bundle By Name(cluster=w1133, "PID Values"=w1132) -> (w1131:T8)
              }
              frame "I (Integral)" {
                n101 = Unbundle By Name(w1139) -> ("PID Values"=w1142:dbl[])
                n102 = Replace Array Subset(array=w1142, new element=w1140, index=1) -> (w1138:dbl[])
                n103 = Bundle By Name(cluster=w1139, "PID Values"=w1138) -> (w1137:T8)
              }
              frame "D (Derivative)" {
                n104 = Unbundle By Name(w1145) -> ("PID Values"=w1148:dbl[])
                n105 = Replace Array Subset(array=w1148, new element=w1146, index=2) -> (w1144:dbl[])
                n106 = Bundle By Name(cluster=w1145, "PID Values"=w1144) -> (w1143:T8)
              }
              frame "Sample Z Step Size (µm)" {
                n107 = Bundle By Name(cluster=w1151, "Z Step Size (µm)"=w1150) -> (w1149:T8)
              }
            }
            n108 = Bundle By Name(cluster=w1109, "Actions"=4Pi_Obj_Lock_-_Actions."Idle") -> (w1108:T8)
            n109 = Send Notification(notification=w1108, notifier=w1111) -> ()  [unwired: 1 in, 2 out]
          }
          event "Sample Z Step No.": Value Change {
            n110 = event-data() -> ("NewVal"=w1153:u32)  [unwired: 1 in]
            n111 = for {
              N: w1153 -> [_]
              tunnel: [w1172] -> w1157 mode=indexing
              tunnel: [w1161] -> w1156 mode=indexing
              i -> [w1171]
              w1162 = T12 3 items=["Grayscale (U8)", "Grayscale (I16)", "Grayscale (SGL)", "Complex (CSG)", "RGB (U32)", "HSL (U32)", "RGB (U64)", "Grayscale (U16)"] ("Image Type")
              w1167 = T12 2 items=["Grayscale (U8)", "Grayscale (I16)", "Grayscale (SGL)", "Complex (CSG)", "RGB (U32)", "HSL (U32)", "RGB (U64)", "Grayscale (U16)"] ("Image Type")
              w1163 = 10 ("Border Size")
              n112 = Number To Decimal String(number=w1171, width (-)=i16 1) -> (decimal integer string=w1169:string)
              n113 = Concatenate Strings("Ref Stack " ("string"), w1169) -> (w1165:string)
              n114 = call "IMAQ Create"("Border Size"=w1163, "Image Name"=w1165, "Image Type"=w1167) -> ("New Image"=w1172:T9)  [unwired: 2 in, 1 out]
              n115 = Concatenate Strings("FFT" ("string"), w1165) -> (w1164:string)
              n116 = call "IMAQ Create"("Border Size"=w1163, "Image Name"=w1164, "Image Type"=w1162) -> ("New Image"=w1161:T9)  [unwired: 2 in, 1 out]
            }
            n117 = Get Notifier Status(notifier=w1155) -> (notifier out=w1159:refnum<notifier>, current notification=w1160:T8)  [unwired: 1 in, 3 out]
            n118 = Bundle By Name(cluster=w1160, "Actions"=4Pi_Obj_Lock_-_Actions."Idle", "Z Step No."=w1153, "Ref Stack (SGL)"=w1157, "Ref FFT Stack (CSG)"=w1156) -> (w1158:T8)
            n119 = Send Notification(notification=w1158, notifier=w1159) -> ()  [unwired: 1 in, 2 out]
          }
          event "Frame Accumulations": Value Change {
            n120 = event-data() -> ("NewVal"=w1175:u16)  [unwired: 1 in]
            n121 = Get Notifier Status(notifier=w1178) -> (notifier out=w1177:refnum<notifier>, current notification=w1176:T8)  [unwired: 1 in, 3 out]
            n122 = Bundle By Name(cluster=w1176, "Actions"=4Pi_Obj_Lock_-_Actions."Idle", "Frame Accumulations"=w1175) -> (w1174:T8)
            n123 = Send Notification(notification=w1174, notifier=w1177) -> ()  [unwired: 1 in, 2 out]
          }
          event "Update Delay (ms)": Value Change {
            n124 = event-data() -> ("NewVal"=w1182:i32)  [unwired: 1 in]
            n125 = Get Notifier Status(notifier=w1185) -> (notifier out=w1184:refnum<notifier>, current notification=w1183:T8)  [unwired: 1 in, 3 out]
            n126 = Bundle By Name(cluster=w1183, "Actions"=4Pi_Obj_Lock_-_Actions."Idle", "Update Delay (ms)"=w1182) -> (w1181:T8)
            n127 = Send Notification(notification=w1181, notifier=w1184) -> ()  [unwired: 1 in, 2 out]
          }
          event "Save Lock Settings": Value Change {
            n128 = event-data() -> ()  [unwired: 1 in, 1 out]
            n129 = Wait on Notification(notifier=w1214) -> (notification=w1212:T8)  [unwired: 3 in, 3 out]
            n130 = Unbundle By Name(w1212) -> ("Z Step Size (µm)"=w1188:dbl, "Z Step No."=w1187:u32, "Z Drift Threshold"=w1211:dbl, "Z Stage Move Limit (µm)"=w1210:dbl, "XY Drift Threshold"=w1209:dbl, "XY Stage Move Limit (µm)"=w1208:dbl, "Frame Accumulations"=w1207:u16, "Abort If Error"=w1206:bool, "Z Correction Active"=w1205:bool, "XY Correction Active"=w1204:bool, "PID Values"=w1194:dbl[])
            n131 = local read "Invert X Axis"() -> (w1192:bool)
            n132 = local read "Invert Y Axis"() -> (w1191:bool)
            n133 = local read "Invert Z Axis"() -> (w1190:bool)
            n134 = local read "Flip XY Axis"() -> (w1193:bool)
            n135 = Bundle By Name(cluster=T7 {"Z Drift Threshold"=0.05, "Z Stage Move Limit (µm)"=1.0, "XY Drift Threshold"=0.05, "XY Stage Move Limit (µm)"=1.0, "Frame Accumulations"=10, "Abort If Error"=FALSE, "Flip XY Axis"=FALSE, "Invert X Axis"=FALSE, "Invert Y Axis"=FALSE, "Invert Z Axis"=FALSE, "Z Correction Active"=TRUE, "XY Correction Active"=TRUE, "PID Values"=[], "Update Delay (ms)"=0, "Sample Z Step Size (µm)"=2.0, "Sample Z Step No."=2, "Z Update Scale Factor"=2.0, "Y Update Scale Factor"=2.0, "X Update Scale Factor"=2.0} ("Lock Settings"), "Sample Z Step Size (µm)"=w1188, "Sample Z Step No."=w1187, "Z Drift Threshold"=w1211, "Z Stage Move Limit (µm)"=w1210, "XY Drift Threshold"=w1209, "XY Stage Move Limit (µm)"=w1208, "Frame Accumulations"=w1207, "Abort If Error"=w1206, "Z Correction Active"=w1205, "XY Correction Active"=w1204, "PID Values"=w1194, "Flip XY Axis"=w1193, "Invert X Axis"=w1192, "Invert Y Axis"=w1191, "Invert Z Axis"=w1190) -> (w1203:T7)
            n136 = control-ref of="This VI"() -> (w1201:refnum<vi>)
            n137 = Flatten To JSON(anything=w1203) -> (JSON string=w1196:string)  [unwired: 2 in, 1 out]
            n138 = property class="VI"(reference=w1201) -> ("Path"=w1198:path)  [unwired: 1 in, 2 out]
            n139 = Strip Path(path=w1198) -> (stripped path=w1197:path)  [unwired: 1 out]
            n140 = Build Path(base path=w1197, name or relative path="4Pi Objective Lock Default Settings") -> (appended path=w1199:path)
            n141 = Build Path(base path=w1199, name or relative path="Default Obj Lock Settings.json") -> (appended path=w1195:path)
            n142 = Write to Text File(file (use dialog)=w1195, text=w1196) -> (refnum out=w1189:refnum<file>)  [unwired: 2 in, 2 out]
            n143 = Close File(refnum=w1189) -> ()  [unwired: 1 in, 2 out]
          }
          event "Start Lock": Value Change {
            n144 = event-data() -> ("NewVal"=w1221:bool)  [unwired: 1 in]
            n145 = Select(t=4Pi_Obj_Lock_-_Actions."Start Lock", s=w1221, f=4Pi_Obj_Lock_-_Actions."Abort" ("Actions")) -> (s? t:f=w1219:T6)
            n146 = Get Notifier Status(notifier=w1224) -> (notifier out=w1223:refnum<notifier>, current notification=w1222:T8)  [unwired: 1 in, 3 out]
            n147 = Bundle By Name(cluster=w1222, "Actions"=w1219, "Running?"=TRUE) -> (w1218:T8)
            n148 = Send Notification(notification=w1218, notifier=w1223) -> ()  [unwired: 1 in, 2 out]
          }
          event "Restart Lock": Value Change {
            n149 = event-data() -> ()  [unwired: 1 in, 1 out]
            n150 = Get Notifier Status(notifier=w1231) -> (notifier out=w1230:refnum<notifier>, current notification=w1229:T8)  [unwired: 1 in, 3 out]
            n151 = Bundle By Name(cluster=w1229, "Actions"=4Pi_Obj_Lock_-_Actions."Restart Lock" ("t")) -> (w1228:T8)
            n152 = local write "Start Lock"(TRUE ("Start Lock")) -> ()
            n153 = Send Notification(notification=w1228, notifier=w1230) -> ()  [unwired: 1 in, 2 out]
          }
          event "Quit": Value Change {
            # "Turn off the OBJ lock before quiting."
            n154 = event-data() -> ("NewVal"=w1242:bool)  [unwired: 1 in]
            n155 = Get Notifier Status(notifier=w1237) -> (notifier out=w1235:refnum<notifier>, current notification=w1233:T8)  [unwired: 1 in, 3 out]
            n156 = Unbundle By Name(w1233) -> ("Running?"=w1236:bool)
            n157 = case shown="True" w1236 {
              tunnel: w1235 -> [w1243 w1247]
              tunnel: [w1243 w1244] -> w1234
              tunnel: w1233 -> [_ w1249]
              frame False {
              }
              frame True {
                n158 = Bundle By Name(cluster=w1249, "Actions"=4Pi_Obj_Lock_-_Actions."Abort") -> (w1246:T8)
                n159 = Send Notification(notification=w1246, notifier=w1247) -> (notifier out=w1245:refnum<notifier>)  [unwired: 1 in, 1 out]
                n160 = while {
                  tunnel: w1245 -> [w1259]
                  tunnel: [w1254] -> w1244
                  i -> [w1253]
                  stop <- w1255 stop-if-true
                  n161 = Get Notifier Status(notifier=w1259) -> (notifier out=w1254:refnum<notifier>, # waiting=w1258:i32)  [unwired: 1 in, 3 out]
                  n162 = Greater?(x=w1253, y=1500) -> (0:w1251:bool)
                  n163 = Less?(x=w1258, y=1) -> (x < y?=w1256:bool)
                  n164 = Or(x=w1256, y=w1251) -> (x .or. y?=w1255:bool)
                  n165 = Wait (ms)(milliseconds to wait=u32 1) -> ()  [unwired: 1 out]
                }
              }
            }
            n166 = Get Notifier Status(notifier=w1234) -> (notifier out=w1239:refnum<notifier>, current notification=w1241:T8)  [unwired: 1 in, 3 out]
            n167 = Bundle By Name(cluster=w1241, "Actions"=4Pi_Obj_Lock_-_Actions."Quit") -> (w1238:T8)
            n168 = Send Notification(notification=w1238, notifier=w1239) -> ()  [unwired: 1 in, 2 out]
          }
        }
      }
      n169 = while {
        tunnel: w197 -> [w223]
        tunnel: w195 -> [w211]
        tunnel: w194 -> [w210]
        tunnel: w196 -> [w222]
        stop <- w218 stop-if-true
        # "Column 1 - Target Lock Values\nColumn 2 - Current Values\nColumn 3 - Differnce Values\nColumn 4 - Initial XYZ Stage Positions"
        n170 = Wait on Notification(notifier=w222, ignore previous (F)=FALSE) -> (notifier out=w217:refnum<notifier>, notification=w220:T8)  [unwired: 2 in, 2 out]
        n171 = Unbundle By Name(w220) -> ("Actions"=w212:T6)
        n172 = Equal?(x=4Pi_Obj_Lock_-_Actions."Quit", y=w212) -> (x = y?=w218:bool)
        n173 = Initialize Array(0.0 ("element"), 3 ("dimension size"), 4 ("dimension size")) -> (w214:dbl[][])
        n174 = while {
          shift-right: [w230] -> _
          shift-left: w212 -> [w238]
          tunnel: w223 -> [w242]
          tunnel: w211 -> [w241]
          tunnel: w210 -> [w240]
          tunnel: w217 -> [w236]
          shift-right: [w224] -> _
          shift-left: w214 -> [w225]
          stop <- w237 stop-if-true
          w232 = 4Pi_Obj_Lock_-_Actions."Abort" ("x")
          n175 = case shown="\"Move XYZ\", \"Move XY\"" w238 {
            selector: w238 -> [_ _ _ _ _ _ _ _ _ _ _ _ _ w794 _ _ _ _ _ _]
            tunnel: w242 -> [_ w263 _ w367 _ _ w478 w512 w556 _ w622 _ _ _ _ _ _ w1033 _ _]
            tunnel: w241 -> [_ w296 _ _ _ _ w454 _ _ _ _ _ w718 w798 _ _ _ _ _ _]
            tunnel: w240 -> [_ w295 w324 w368 _ w428 w453 _ _ _ _ _ w717 _ w876 _ _ _ _ _]
            tunnel: FALSE -> [w245 w308 w320 w366 w406 w424 w481 w543 w558 w595 w652 w700 w724 w824 w881 w1008 w1020 w1037 _ _]
            tunnel: [4Pi_Obj_Lock_-_Actions."Exit Loop" ("x") w265 4Pi_Obj_Lock_-_Actions."Get Ref Stack" ("x") w371 4Pi_Obj_Lock_-_Actions."Move To Init Z" ("x") 4Pi_Obj_Lock_-_Actions."Get Initial Position" ("x") w473 w526 w561 4Pi_Obj_Lock_-_Actions."Get Current Position" ("x") w639 w678 w728 w813 w857 4Pi_Obj_Lock_-_Actions."Delay" ("x") 4Pi_Obj_Lock_-_Actions."Get Current Z Position" ("x") 4Pi_Obj_Lock_-_Actions."Exit Loop" ("x") 4Pi_Obj_Lock_-_Actions."Exit Loop" ("x") 4Pi_Obj_Lock_-_Actions."Quit" ("x")] -> w231
            tunnel: [w245 w308 w320 w366 w406 w424 w481 w543 w558 w595 w652 w700 w724 w824 w881 w1008 w1020 w1037 TRUE TRUE] -> w237
            tunnel: w236 -> [w244 w279 w325 w370 w411 w422 w480 w542 w568 w617 w651 w699 w759 w823 w879 w1006 w1018 w1041 w1047 w1051]
            tunnel: [w244 w274 w323 w369 w408 w422 w480 w534 w567 w593 w650 w698 w727 w822 w878 w1005 w1014 w1040 w1047 w1050] -> w235
            tunnel: w225 -> [w243 w292 w319 w365 w405 w423 w466 w541 w557 w594 w627 w688 w723 w784 w855 w987 w1017 w1036 w1046 w1059]
            tunnel: [w243 w291 w319 w365 w405 w423 w465 w540 w557 w594 w626 w685 w723 w784 w855 w987 w1017 w1036 w1046 w1059] -> w224
            frame "Idle", Default {
            }
            frame "Start Lock" {
              w248 = T18 [] ("History Data")
              w288 = FALSE ("Move Limit Error")
              w293 = Stage_Actions."Get Position" ("Actions")
              n176 = control-ref of="This VI"() -> (w306:refnum<vi>)
              n177 = call "Stages Messenger.vi"("Stage Notifier Name"=w296, "Actions"=w293) -> ("Positions"=w297:dbl[])  [unwired: 9 in, 4 out]
              n178 = call "Stages Messenger.vi"("Stage Notifier Name"=w295, "Actions"=w293) -> ("Positions"=w298:dbl[])  [unwired: 9 in, 4 out]
              n179 = property class="VI"(reference=w306) -> ("Path"=w303:path)  [unwired: 1 in, 2 out]
              n180 = local write "Move Limit Error"(w288) -> ()
              n181 = local write "Fit Error"(w288) -> ()
              n182 = Index Array(array=w298, index=0) -> (element=w294:dbl)
              n183 = Strip Path(path=w303) -> (stripped path=w302:path)  [unwired: 1 out]
              n184 = Build Path(base path=w302, name or relative path="4Pi Objective Lock Default Settings") -> (appended path=w304:path)
              n185 = Build Array (concatenate)(w297, w294) -> (w273:dbl[])
              n186 = Build Path(base path=w304, name or relative path="Initial Stage Positions.json") -> (appended path=w300:path)
              n187 = Flatten To JSON(anything=w273) -> (JSON string=w301:string)  [unwired: 2 in, 1 out]
              n188 = Replace Array Subset(array=w292, new element=w273, index (col)=3 ("disabled index (col)")) -> (w291:dbl[][])  [unwired: 1 in]
              n189 = Index Array(array=w273, index #1=0 ("index"), index #2=1 ("index"), index #3=2 ("index")) -> (element #1=w269:dbl, element #2=w267:dbl, element #3=w268:dbl)
              n190 = Write to Text File(file (use dialog)=w300, text=w301) -> (refnum out=w289:refnum<file>)  [unwired: 2 in, 2 out]
              n191 = local write "X Axis Position (µm)"(w269) -> ()
              n192 = local write "Y Axis Position (µm)"(w267) -> ()
              n193 = local write "Z Axis Position (µm)"(w268) -> ()
              n194 = Get Notifier Status(notifier=w279) -> (notifier out=w274:refnum<notifier>, current notification=w278:T8)  [unwired: 1 in, 3 out]
              n195 = Close File(refnum=w289) -> ()  [unwired: 1 in, 2 out]
              n196 = Unbundle By Name(w278) -> ("Cur Image (SGL)"=w277:T9)
              n197 = Unbundle By Name(w278) -> ("Z Step No."=w276:u32, "Ref Stack (SGL)"=w275:T9[])
              n198 = call "Camera Messenger.vi"("Notifier Name"=w263, "General Camera Actions"=Generic_Camera_Actions."Get ROI", "Camera ROI"=T14 {"H_Offset"=0, "V_Offset"=0, "H_Width"=0, "V_Width"=0} ("General Camera ROI")) -> ("Notifier Name Dup"=w260:string, "Camera ROI"=w280:T14)  [unwired: 7 in, 4 out]
              n199 = Unbundle By Name(w280) -> ("H_Width"=w285:u16, "V_Width"=w283:u16)
              n200 = To Long Integer(number=w285) -> (32bit integer=w284:i32)
              n201 = To Long Integer(number=w283) -> (32bit integer=w282:i32)
              n202 = Initialize Array(sgl 0.0 ("element"), w284, w282) -> (w249:sgl[][])
              n203 = for {
                N: w276 -> [_]
                tunnel: w249 -> [w317]
                tunnel: w275 -> [w318] mode=indexing
                n204 = call "IMAQ ArrayToImage"("Image Pixels (Float)"=w317, "Image"=w318) -> ()  [unwired: 8 in, 2 out]
              }
              n205 = call "IMAQ ArrayToImage"("Image Pixels (Float)"=w249, "Image"=w277) -> ()  [unwired: 8 in, 2 out]
              n206 = Array Size(array=w249) -> (size(s)=w255:i32[])
              n207 = To Double Precision Float(number=w255) -> (double precision float=w258:dbl[])
              n208 = call "Camera Messenger.vi"("Notifier Name"=w260, "General Camera Actions"=Generic_Camera_Actions."Live Preview") -> ("Notifier Name Dup"=w261:string)  [unwired: 8 in, 5 out]
              n209 = Divide(x=w258, y=2.0 ("index")) -> (x/y=w256:dbl[])
              n210 = while {
                tunnel: w261 -> [w315]
                tunnel: [w310] -> w259
                i -> [w314]
                stop <- w311 stop-if-true
                n211 = call "Camera Messenger.vi"("Notifier Name"=w315, "General Camera Actions"=Generic_Camera_Actions."Status") -> ("Running?"=w312:bool)  [unwired: 8 in, 5 out]
                n212 = Greater?(x=w314, y=3000) -> (0:w310:bool)
                n213 = Or(x=w312, y=w310) -> (x .or. y?=w311:bool)
                n214 = Wait (ms)(milliseconds to wait=u32 1) -> ()  [unwired: 1 out]
              }
              n215 = Round Toward -Infinity(1:w256) -> (0:w254:dbl[])
              n216 = Index Array(array=w254, index #1=0 ("index"), index #2=1 ("index")) -> (element #1=→"Target Y Position cc (px)":dbl, element #2=→"Target X Position cc (px)":dbl)
              n217 = Select(t=4Pi_Obj_Lock_-_Actions."Exit Loop", s=w259, f=4Pi_Obj_Lock_-_Actions."Get Target Z Position" ("x")) -> (s? t:f=w265:T6)
              n218 = property on="X Target and Fit Position (µm)" class="WFChart (strict)"("History Data"=w248) -> ()  [unwired: 2 in, 2 out]
              n219 = property on="Y Target and Fit Position (µm)" class="WFChart (strict)"("History Data"=w248) -> ()  [unwired: 2 in, 2 out]
              n220 = property on="Z Target and Fit Value (µm)" class="WFChart (strict)"("History Data"=w248) -> ()  [unwired: 2 in, 2 out]
              n221 = property on="CC Max" class="WFChart (strict)"("History Data"=cluster{"pixel size (µm)":dbl}[] []) -> ()  [unwired: 2 in, 2 out]
            }
            frame "Get Target Z Position" {
              w346 = 0.0 ("Target Z (µm)")
              n222 = Get Notifier Status(notifier=w325) -> (notifier out=w344:refnum<notifier>, current notification=w349:T8)  [unwired: 1 in, 3 out]
              n223 = Unbundle By Name(w349) -> ("Z Step No."=w342:u32, "Z Step Size (µm)"=w341:dbl, "Z Stage Move Limit (µm)"=w339:dbl)
              n224 = Unbundle By Name(w349) -> ("Z Step No."=w334:u32, "Z Step Size (µm)"=w347:dbl)
              n225 = Divide(x=w342, y=2.0) -> (x/y=w332:dbl)
              n226 = Round Toward -Infinity(1:w332) -> (0:w331:dbl)
              n227 = Multiply(x=w331, y=w341) -> (x*y=w336:dbl)
              n228 = Decrement(x=w334) -> (x-1=w333:u32)
              n229 = Negate(x=w336) -> (-x=w335:dbl)
              n230 = Negate(x=w339) -> (-x=w340:dbl)
              n231 = In Range and Coerce(upper limit=w339, x=w335, lower limit=w340) -> (coerced(x)=w337:dbl)  [unwired: 1 out]
              n232 = Add(x=w346, y=w337) -> (x+y=w338:dbl)
              n233 = Build Array(w338) -> (w348:dbl[])
              n234 = for {
                N: w333 -> [_]
                tunnel: w347 -> [w360]
                shift-right: [w361] -> w345
                shift-left: w348 -> [w362]
                shift-right: [w358] -> _
                shift-left: w338 -> [w359]
                n235 = Add(x=w359, y=w360) -> (x+y=w358:dbl)
                n236 = Build Array (concatenate)(w362, w358) -> (w361:dbl[])
              }
              n237 = Build Array(w337) -> (w350:dbl[])
              n238 = call "Stages Messenger.vi"("Stage Notifier Name"=w324, "Actions"=Stage_Actions."MVR", "Setpoint"=w350, "Axis"=bool[] [TRUE], "Exit While Busy?"=FALSE) -> ("Stage Notifier Name (Dup)"=w329:string, "Status"=w330:T19)  [unwired: 6 in, 3 out]
              n239 = case shown="Default" w330 {
                tunnel: [w356] -> w328
                tunnel: w329 -> [w356]
                frame Default {
                  n240 = Wait (ms)(milliseconds to wait=u32 150) -> ()  [unwired: 1 out]
                }
              }
              n241 = Bundle By Name(cluster=w349, "Sample Z (µm)"=w345) -> (w343:T8)
              n242 = call "Stages Messenger.vi"("Stage Notifier Name"=w328, "Actions"=Stage_Actions."Get Position") -> ("Positions"=w326:dbl[])  [unwired: 9 in, 4 out]
              n243 = Index Array(array=w326, index=0) -> (element=w321:dbl)
              n244 = Send Notification(notification=w343, notifier=w344) -> (notifier out=w323:refnum<notifier>)  [unwired: 1 in, 1 out]
              n245 = local write "Z Axis Position (µm)"(w321) -> ()
              "Target Z (µm)" <- w346
            }
            frame "Get Ref Stack" {
              n246 = Get Notifier Status(notifier=w370) -> (notifier out=w369:refnum<notifier>, current notification=w364:T8)  [unwired: 1 in, 3 out]
              n247 = Unbundle By Name(w364) -> ("Z Step No."=w374:u32, "Ref Stack (SGL)"=w373:T9[])
              n248 = Unbundle By Name(w364) -> ("Frame Accumulations"=w363:u16)
              n249 = Unbundle By Name(w364) -> ("Z Step Size (µm)"=w372:dbl)
              n250 = while {
                tunnel: w367 -> [w392]
                tunnel: w374 -> [w389]
                tunnel: w369 -> [w391]
                tunnel: [w381] -> w371
                tunnel: w373 -> [w380] mode=indexing
                tunnel: w372 -> [w379]
                tunnel: w368 -> [w378]
                tunnel: w363 -> [w375]
                i -> [w388]
                stop <- w384 stop-if-true
                n251 = flat-sequence {
                  tunnel: w392 -> [w395]
                  tunnel: w380 -> [w393]
                  tunnel: w375 -> [w394]
                  tunnel: w379 -> [w399]
                  tunnel: w378 -> [w398]
                  frame #0 {
                    n252 = call "Generic Camera Get New Camera Image.vi"("Camera Notifier Name"=w395, "Frames"=w394) -> ("Image - U16"=w397:u16[][])  [unwired: 11 in, 2 out]
                    n253 = To Single Precision Float(number=w397) -> (single precision float=w396:sgl[][])
                    n254 = call "IMAQ ArrayToImage"("Image Pixels (Float)"=w396, "Image"=w393) -> ()  [unwired: 8 in, 2 out]
                  }
                  frame #1 {
                    n255 = Build Array(w399) -> (w403:dbl[])
                    n256 = call "Stages Messenger.vi"("Stage Notifier Name"=w398, "Actions"=Stage_Actions."MVR", "Setpoint"=w403, "Axis"=bool[] [TRUE], "Exit While Busy?"=FALSE) -> ()  [unwired: 6 in, 5 out]
                  }
                  frame #2 {
                    n257 = Wait (ms)(milliseconds to wait=u32 150) -> ()  [unwired: 1 out]
                  }
                }
                n258 = Get Notifier Status(notifier=w391) -> (current notification=w383:T8)  [unwired: 1 in, 4 out]
                n259 = To Unsigned Long Integer(number=w388) -> (unsigned 32bit integer=w387:u32)
                n260 = Increment(x=w387) -> (x+1=w390:u32)
                n261 = Unbundle By Name(w383) -> ("Running?"=w386:bool)
                n262 = Greater Or Equal?(x=w390, y=w389) -> (x >= y?=w385:bool)
                n263 = Not(x=w386) -> (.not. x?=w382:bool)
                n264 = Or(x=w382, y=w385) -> (x .or. y?=w384:bool)
                n265 = Select(t=4Pi_Obj_Lock_-_Actions."Abort" ("x"), s=w382, f=4Pi_Obj_Lock_-_Actions."Cal Ref FFT") -> (s? t:f=w381:T6)
              }
            }
            frame "Cal Ref FFT" {
              n266 = Get Notifier Status(notifier=w411) -> (notifier out=w408:refnum<notifier>, current notification=w412:T8)  [unwired: 1 in, 3 out]
              n267 = Unbundle By Name(w412) -> ("Ref Stack (SGL)"=w410:T9[], "Ref FFT Stack (CSG)"=w409:T9[])
              n268 = for {
                tunnel: w410 -> [w414] mode=indexing
                tunnel: w409 -> [w413] mode=indexing
                n269 = call "4Pi Obj Lock - Norm FFT.vi"("FFT Image Dst"=w413, "Image In"=w414) -> ()  [unwired: 8 in, 2 out]
              }
            }
            frame "Move To Init Z" {
              # "initial z stage position"
              n270 = Index Array(array=w423, index (row)=2, index (col)=3 ("disabled index (col)")) -> (element=w425:dbl)
              n271 = flat-sequence {
                tunnel: w428 -> [w438]
                tunnel: [w437] -> w430
                tunnel: w425 -> [w433]
                tunnel: [w431] -> w429
                tunnel: w430 -> [w442]
                tunnel: w429 -> [w441]
                tunnel: [w440] -> w415
                tunnel: [w447] -> w417
                tunnel: w415 -> [w447]
                frame #0 {
                  n272 = call "Stages Messenger.vi"("Stage Notifier Name"=w438, "Actions"=Stage_Actions."Get Position") -> ("Stage Notifier Name (Dup)"=w437:string, "Positions"=w435:dbl[])  [unwired: 9 in, 3 out]
                  n273 = Index Array(array=w435, index=0) -> (element=w434:dbl)
                  n274 = Subtract(x=w433, y=w434) -> (x-y=w432:dbl)
                  n275 = Build Array(w432) -> (w431:dbl[])
                }
                frame #1 {
                  n276 = call "Stages Messenger.vi"("Stage Notifier Name"=w442, "Actions"=Stage_Actions."MVR", "Setpoint"=w441, "Axis"=bool[] [TRUE], "Exit While Busy?"=FALSE) -> ("Stage Notifier Name (Dup)"=w440:string)  [unwired: 6 in, 4 out]
                }
                frame #2 {
                  n277 = Wait (ms)(milliseconds to wait=u32 150) -> ()  [unwired: 1 out]
                }
              }
              n278 = call "Stages Messenger.vi"("Stage Notifier Name"=w417, "Actions"=Stage_Actions."Get Position") -> ("Positions"=w419:dbl[])  [unwired: 9 in, 4 out]
              n279 = Index Array(array=w419, index=0) -> (element=w418:dbl)
              n280 = local write "Z Axis Position (µm)"(w418) -> ()
            }
            frame "Restart Lock" {
              w448 = T18 [] ("History Data")
              w449 = FALSE ("Move Limit Error")
              # "Make sure the camera is running, if not abort."
              n281 = control-ref of="This VI"() -> (w471:refnum<vi>)
              n282 = call "Camera Messenger.vi"("Notifier Name"=w478, "General Camera Actions"=Generic_Camera_Actions."Live Preview") -> ("Notifier Name Dup"=w477:string)  [unwired: 8 in, 5 out]
              n283 = property class="VI"(reference=w471) -> (error out=w457:errorcluster, "Path"=w468:path)  [unwired: 1 in, 1 out]
              n284 = while {
                tunnel: w477 -> [w507]
                tunnel: [w502] -> w476
                i -> [w506]
                stop <- w503 stop-if-true
                n285 = call "Camera Messenger.vi"("Notifier Name"=w507, "General Camera Actions"=Generic_Camera_Actions."Status") -> ("Running?"=w504:bool)  [unwired: 8 in, 5 out]
                n286 = Greater?(x=w506, y=3000) -> (0:w502:bool)
                n287 = Or(x=w504, y=w502) -> (x .or. y?=w503:bool)
                n288 = Wait (ms)(milliseconds to wait=u32 1) -> ()  [unwired: 1 out]
              }
              n289 = Strip Path(path=w468) -> (stripped path=w467:path)  [unwired: 1 out]
              n290 = Build Path(base path=w467, name or relative path="4Pi Objective Lock Default Settings") -> (appended path=w469:path)
              n291 = Build Path(base path=w469, name or relative path="Initial Stage Positions.json") -> (appended path=w463:path)
              n292 = Read from Text File(file (use dialog)=w463, error in=w457) -> (refnum out=w462:refnum<file>, text=w461:string, error out=w460:errorcluster)  [unwired: 2 in, 1 out]
              n293 = Close File(refnum=w462, error in=w460) -> (error out=w459:errorcluster)  [unwired: 1 out]
              n294 = local write "Move Limit Error"(w449) -> ()
              n295 = local write "Fit Error"(w449) -> ()
              n296 = Unflatten From JSON(JSON string=w461, type and defaults=dbl[] [], error in (no error)=w459) -> (value=w455:dbl[], error out=w456:errorcluster)  [unwired: 4 in]
              n297 = case shown="Error" w456 {
                tunnel: w455 -> [w483 _]
                tunnel: w454 -> [w490 w495]
                tunnel: w453 -> [w489 w494]
                tunnel: [w483 w493] -> w452
                tunnel: u32 150 ("milliseconds to wait") -> [w482 w492]
                tunnel: [w482 w492] -> w450
                frame No Error {
                  w491 = Stage_Actions."MOVE" ("Actions")
                  n298 = Split 1D Array(array=w483, index=2) -> (first subarray=w487:dbl[], second subarray=w486:dbl[])
                  n299 = call "Stages Messenger.vi"("Stage Notifier Name"=w490, "Actions"=w491, "Setpoint"=w487, "Axis"=bool[] [TRUE, TRUE]) -> ()  [unwired: 7 in, 5 out]
                  n300 = call "Stages Messenger.vi"("Stage Notifier Name"=w489, "Actions"=w491, "Setpoint"=w486, "Axis"=bool[] [TRUE]) -> ()  [unwired: 7 in, 5 out]
                }
                frame Error {
                  w496 = Stage_Actions."Get Position" ("Actions")
                  n301 = call "Stages Messenger.vi"("Stage Notifier Name"=w495, "Actions"=w496) -> ("Positions"=w498:dbl[])  [unwired: 9 in, 4 out]
                  n302 = call "Stages Messenger.vi"("Stage Notifier Name"=w494, "Actions"=w496) -> ("Positions"=w499:dbl[])  [unwired: 9 in, 4 out]
                  n303 = Index Array(array=w499, index=0) -> (element=w497:dbl)
                  n304 = Build Array (concatenate)(w498, w497) -> (w493:dbl[])
                }
              }
              n305 = Wait (ms)(milliseconds to wait=w450) -> ()  [unwired: 1 out]
              n306 = Replace Array Subset(array=w466, new element=w452, index (col)=3 ("disabled index (col)")) -> (w465:dbl[][])  [unwired: 1 in]
              n307 = property on="X Target and Fit Position (µm)" class="WFChart (strict)"("History Data"=w448) -> ()  [unwired: 2 in, 2 out]
              n308 = property on="Y Target and Fit Position (µm)" class="WFChart (strict)"("History Data"=w448) -> ()  [unwired: 2 in, 2 out]
              n309 = property on="Z Target and Fit Value (µm)" class="WFChart (strict)"("History Data"=w448) -> ()  [unwired: 2 in, 2 out]
              n310 = Select(t=4Pi_Obj_Lock_-_Actions."Exit Loop" ("x"), s=w476, f=4Pi_Obj_Lock_-_Actions."Get Initial Position" ("x")) -> (s? t:f=w473:T6)
            }
            frame "Get Initial Position" {
              w519 = 0 ("index")
              # "Set target values"
              n311 = Get Notifier Status(notifier=w542) -> (notifier out=w535:refnum<notifier>, current notification=w511:T8)  [unwired: 1 in, 3 out]
              n312 = Unbundle By Name(w511) -> ("Frame Accumulations"=w510:u16)
              n313 = Bundle By Name(cluster=w511, "Running?"=TRUE) -> (w532:T8)
              n314 = Send Notification(notification=w532, notifier=w535) -> (notifier out=w534:refnum<notifier>)  [unwired: 1 in, 1 out]
              n315 = call "Generic Camera Get New Camera Image.vi"("Camera Notifier Name"=w512, "Frames"=w510) -> ("Image - U16"=w509:u16[][])  [unwired: 11 in, 2 out]
              n316 = call "2D Gaussian - Fit Image U16.vi"("Image In (U16)"=w509) -> ("Best Fit Params"=w539:T20, "Error Out"=w525:errorcluster)  [unwired: 13 in]
              n317 = Unbundle By Name(w525) -> ("status"=w524:bool)
              n318 = Cluster To Array(cluster=w539) -> (array=w538:dbl[])
              n319 = local write "Fit Error"(w524) -> ()
              n320 = Array Subset(array=w538, index=1, length=4) -> (w531:dbl[])
              n321 = Index Array(array=w531, index #1=0 ("index"), index #2=1 ("index"), index #3=2 ("index"), index #4=3 ("index")) -> (element #1=w513:dbl, element #2=w514:dbl, element #3=w521:dbl, element #4=w520:dbl)
              "Target X Position (px)" <- w513
              "Target Y Position (px)" <- w514
              n322 = Divide(x=w521, y=w520) -> (x/y=w515:dbl)
              "Target sx/sy" <- w515
              n323 = Replace Array Subset(array=w541, new element #1=w513, index (row) #1=0 ("disabled index (row)"), index (col) #1=w519, new element #2=w514, index (row) #2=1 ("disabled index (row)"), index (col) #2=w519, new element #3=w515, index (row) #3=2 ("disabled index (row)"), index (col) #3=w519) -> (w540:dbl[][])
              n324 = Select(t=4Pi_Obj_Lock_-_Actions."Abort" ("x"), s=w524, f=4Pi_Obj_Lock_-_Actions."Get Current Z Position" ("x")) -> (s? t:f=w526:T6)
            }
            frame "Get Current Z Position" {
              n325 = Get Notifier Status(notifier=w568) -> (notifier out=w567:refnum<notifier>, current notification=w555:T8)  [unwired: 1 in, 3 out]
              n326 = Unbundle By Name(w555) -> ("CC Image (SGL)"=w546:T9, "CC Image Max (SGL)"=w545:T9)
              n327 = Unbundle By Name(w555) -> ("Ref FFT Stack (CSG)"=w574:T9[])
              n328 = Unbundle By Name(w555) -> ("Cur Image (SGL)"=w551:T9, "Tmp Image FFT (CSG)"=w564:T9[])
              n329 = Unbundle By Name(w555) -> ("Sample Z (µm)"=w576:dbl[])
              n330 = Unbundle By Name(w555) -> ("Frame Accumulations"=w554:u16)
              n331 = call "Generic Camera Get New Camera Image.vi"("Camera Notifier Name"=w556, "Frames"=w554) -> ("Image - U16"=w553:u16[][])  [unwired: 11 in, 2 out]
              n332 = Index Array(array=w564, index #1=0 ("index"), index #2=1 ("index"), index #3=2 ("index")) -> (element #1=w562:T9, element #2=w548:T9, element #3=w547:T9)
              n333 = To Single Precision Float(number=w553) -> (single precision float=w550:sgl[][])
              n334 = call "IMAQ ArrayToImage"("Image Pixels (Float)"=w550, "Image"=w551) -> ("Image Out"=w552:T9)  [unwired: 8 in, 1 out]
              n335 = call "4Pi Obj Lock - Norm FFT.vi"("FFT Image Dst"=w562, "Image In"=w552) -> ("FFT Image Out"=w572:T9)  [unwired: 8 in, 1 out]
              n336 = call "IMAQ ComplexConjugate"("Image Src"=w572) -> ("Image Dst Out"=w571:T9)  [unwired: 3 in, 1 out]
              n337 = for {
                tunnel: [w581] -> w577 mode=indexing
                tunnel: w571 -> [w587]
                tunnel: w574 -> [w586] mode=indexing
                shift-right: [w581] -> _
                shift-left: sgl 0.0 ("Max CC") -> [w582]
                tunnel: w548 -> [w585]
                tunnel: w547 -> [w584]
                tunnel: w546 -> [w580]
                tunnel: w545 -> [w578]
                n338 = call "4Pi Obj Lock - Get Cross Correlation.vi"("Ref FFT image"=w586, "Cur FFT Image"=w587, "FFT CC image"=w585, "iFFT image"=w584, "CC image"=w580) -> ("Max CC"=w581:sgl, "CC image Out"=w579:T9)  [unwired: 8 in, 1 out]
                n339 = Greater?(x=w581, y=w582) -> (0:w583:bool)
                n340 = case shown="True" w583 {
                  tunnel: w579 -> [_ w589]
                  tunnel: w578 -> [_ w588]
                  frame False {
                  }
                  frame True {
                    n341 = call "IMAQ Copy"("Image Dst"=w588, "Image Src"=w589) -> ()  [unwired: 4 in, 2 out]
                  }
                }
              }
              n342 = To Double Precision Float(number=w577) -> (double precision float=w573:dbl[])
              n343 = call "4Pi Obj Lock - Find Peak Position.vi"("Fit Size"=2, "y"=w573, "x"=w576) -> ("Peak value"=→"CC Max Value":dbl, "Coerced Peak Position"=w570:dbl)  [unwired: 6 in, 1 out]
              "Measured Z (µm)" <- w570
              n344 = Not A Number/Path/Refnum?(number/path/refnum=w570) -> (NaN/Path/Refnum?=w569:bool)
              n345 = Select(t=4Pi_Obj_Lock_-_Actions."Get Current Z Position" ("x"), s=w569, f=4Pi_Obj_Lock_-_Actions."Get Current XY Position") -> (s? t:f=w561:T6)
            }
            frame "Get Current XY Position" {
              w605 = 3 ("edge size")
              n346 = Get Notifier Status(notifier=w617) -> (notifier out=w593:refnum<notifier>, current notification=w616:T8)  [unwired: 1 in, 3 out]
              n347 = Unbundle By Name(w616) -> ("CC Image Max (SGL)"=w615:T9)
              n348 = call "IMAQ ImageToArray"("Image"=w615) -> ("Image Pixels (Float)"=w602:sgl[][])  [unwired: 3 in, 4 out]
              n349 = call "4Pi Obj Lock - FFT shift 2D.vi"("Input image"=w602) -> ("fft shifted image"=w601:sgl[][])  [unwired: 10 in]
              n350 = call "4Pi Obj Lock - Crop Imag at Max.vi"("edge size"=w605, "Input array"=w601) -> ("Y"=w611:i32, "X"=w612:i32, "subarray"=w614:sgl[][])  [unwired: 6 in, 1 out]
              n351 = To Double Precision Float(number=w614) -> (double precision float=w591:dbl[][])
              n352 = Build Array(w612, w611) -> (w610:i32[])
              n353 = call "2D Gaussian - Fit -init.vi"("Image In (DBL)"=w591, "width"=10.0) -> ("Best Fit Params"=w613:T20)  [unwired: 12 in, 1 out]
              n354 = To Double Precision Float(number=w610) -> (double precision float=w607:dbl[])
              n355 = Unbundle By Name(w613) -> ("X Position"=w609:dbl, "Y Position"=w608:dbl)
              n356 = Build Array(w609, w608) -> (w606:dbl[])
              n357 = To Double Precision Float(number=w605) -> (double precision float=w604:dbl)
              n358 = Subtract(x=w606, y=w604) -> (x-y=w603:dbl[])
              n359 = Add(x=w603, y=w607) -> (x+y=w598:dbl[])
              n360 = Index Array(array=w598, index #1=0 ("index"), index #2=1 ("index")) -> (element #1=→"Measured X Position cc (px)":dbl, element #2=→"Measured Y Position cc (px)":dbl)
            }
            frame "Get Current Position" {
              w631 = 1 ("index")
              # "retake current image"
              # "Update current values"
              n361 = Get Notifier Status(notifier=w651) -> (notifier out=w650:refnum<notifier>, current notification=w619:T8)  [unwired: 1 in, 3 out]
              n362 = Unbundle By Name(w619) -> ("Abort If Error"=w644:bool, "Cur Image (SGL)"=w621:T9)
              n363 = case shown="True" TRUE {
                tunnel: w622 -> [_ w661]
                tunnel: w621 -> [w655 w658]
                tunnel: w619 -> [_ w660]
                tunnel: [w653 w657] -> w618
                frame False {
                  n364 = call "IMAQ ImageToArray"("Image"=w655) -> ("Image Pixels (Float)"=w654:sgl[][])  [unwired: 3 in, 4 out]
                  n365 = To Unsigned Word Integer(number=w654) -> (unsigned 16bit integer=w653:u16[][])
                }
                frame True {
                  n366 = Unbundle By Name(w660) -> ("Frame Accumulations"=w659:u16)
                  n367 = call "Generic Camera Get New Camera Image.vi"("Camera Notifier Name"=w661, "Frames"=w659) -> ("Image - U16"=w657:u16[][])  [unwired: 11 in, 2 out]
                  n368 = To Single Precision Float(number=w657) -> (single precision float=w656:sgl[][])
                  n369 = call "IMAQ ArrayToImage"("Image Pixels (Float)"=w656, "Image"=w658) -> ()  [unwired: 8 in, 2 out]
                }
              }
              n370 = call "2D Gaussian - Fit Image U16.vi"("Image In (U16)"=w618) -> ("Best Fit Params"=w649:T20, "Error Out"=w645:errorcluster)  [unwired: 13 in]
              n371 = Unbundle By Name(w645) -> ("status"=w643:bool)
              "Fit Error" <- w643
              n372 = And(x=w644, y=w643) -> (x .and. y?=w642:bool)
              n373 = Cluster To Array(cluster=w649) -> (array=w648:dbl[])
              n374 = Array Subset(array=w648, index=1, length=4) -> (w632:dbl[])
              n375 = Index Array(array=w632, index #1=0 ("index"), index #2=1 ("index"), index #3=2 ("index"), index #4=3 ("index")) -> (element #1=w623:dbl, element #2=w624:dbl, element #3=w634:dbl, element #4=w633:dbl)
              "Measured X Position (px)" <- w623
              "Measured Y Position (px)" <- w624
              n376 = Divide(x=w634, y=w633) -> (x/y=w625:dbl)
              "Measured sx/sy" <- w625
              n377 = Select(t=4Pi_Obj_Lock_-_Actions."Abort" ("x"), s=w642, f=4Pi_Obj_Lock_-_Actions."Check Drift" ("x")) -> (s? t:f=w639:T6)
              n378 = Replace Array Subset(array=w627, new element #1=w623, index (row) #1=0 ("disabled index (row)"), index (col) #1=w631, new element #2=w624, index (row) #2=1 ("disabled index (row)"), index (col) #2=w631, new element #3=w625, index (row) #3=2 ("disabled index (row)"), index (col) #3=w631) -> (w626:dbl[][])
            }
            frame "Check Drift" {
              # "Update the PID difference between target values and current values"
              # "Check if Sigma X / Sigma Y is over the limit"
              # "Check if XY values are over the limit"
              n379 = Get Notifier Status(notifier=w699) -> (notifier out=w698:refnum<notifier>, current notification=w697:T8)  [unwired: 1 in, 3 out]
              n380 = Unbundle By Name(w697) -> ("Z Correction Active"=w674:bool, "XY Correction Active"=w676:bool, "XY Drift Threshold"=w668:dbl, "Z Drift Threshold"=w664:dbl, "PID Values"=w696:dbl[])
              n381 = Index Array(array=w688, index (col) #1=0 ("disabled index (col)"), index (col) #2=1 ("index (col)")) -> (element #1=w690:dbl[], element #2=w689:dbl[])  [unwired: 2 in]
              n382 = local read "Metric scale sx/sy"() -> (w662:dbl)
              n383 = Array To Cluster(array=w696) -> (cluster=w670:T21)
              n384 = local read "pixel size (µm)"() -> (w667:dbl)
              n385 = Build Array(w670) -> (w695:T22)
              n386 = Divide(x=w668, y=w667) -> (x/y=w669:dbl)
              n387 = Divide(x=w664, y=w662) -> (x/y=w663:dbl)
              n388 = call-poly <vilib>:"PID.vi"("PID gains"=w695, "process variable"=w689, "setpoint"=w690) -> ("dt out (s)"=w665:dbl, "output"=w686:dbl[])  [unwired: 7 in]
              n389 = Build Array(w669, w669, w663) -> (w693:dbl[])
              n390 = local write "dt z (s)"(w665) -> ()
              n391 = Replace Array Subset(array=w688, new element=w686, index (col)=2 ("disabled index (col)")) -> (w685:dbl[][])  [unwired: 1 in]
              n392 = Absolute Value(x=w686) -> (abs(x)=w694:dbl[])
              n393 = Greater?(x=w694, y=w693) -> (0:w684:bool[])
              n394 = Split 1D Array(array=w684, index=2) -> (first subarray=w682:bool[], second subarray=w681:bool[])
              n395 = Or Array Elements(Boolean array=w682) -> (logical OR=w677:bool)
              n396 = Or Array Elements(Boolean array=w681) -> (logical OR=w666:bool)
              n397 = And(x=w676, y=w677) -> (x .and. y?=w675:bool)
              n398 = And(x=w674, y=w666) -> (x .and. y?=w673:bool)
              n399 = Build Array(w675, w673) -> (w680:bool[])
              n400 = Boolean Array To Number(Boolean array=w680) -> (number=w679:u32)
              n401 = case shown="3" w679 {
                tunnel: [4Pi_Obj_Lock_-_Actions."Update Plots" ("x") 4Pi_Obj_Lock_-_Actions."Move XY" ("x") 4Pi_Obj_Lock_-_Actions."Move Z" ("x") 4Pi_Obj_Lock_-_Actions."Move XYZ" ("x")] -> w678
                tunnel: [w701 TRUE FALSE w709] -> w672
                tunnel: [w701 FALSE TRUE w709] -> w671
                frame 0, Default {
                  w701 = FALSE
                  # "XYZ within limits, no move"
                }
                frame 1 {
                  # "X or Y outside limit, move XY"
                }
                frame 2 {
                  # "Sigma X / Y outside limit, move Z"
                }
                frame 3 {
                  w709 = TRUE
                  # "XYZ outside limit, move all"
                }
              }
              "XY Move" <- w672
              "Z Move" <- w671
            }
            frame "Check Drift cc" {
              w719 = Stage_Actions."Get Position" ("Actions")
              n402 = Get Notifier Status(notifier=w759) -> (notifier out=w727:refnum<notifier>, current notification=w745:T8)  [unwired: 1 in, 3 out]
              n403 = call "Stages Messenger.vi"("Stage Notifier Name"=w718, "Actions"=w719) -> ("Positions"=w716:dbl[])  [unwired: 9 in, 4 out]
              n404 = call "Stages Messenger.vi"("Stage Notifier Name"=w717, "Actions"=w719) -> ("Positions"=w720:dbl[])  [unwired: 9 in, 4 out]
              n405 = Index Array(array=w716, index #1=0 ("index"), index #2=1 ("index")) -> (element #1=w711:dbl, element #2=w712:dbl)
              n406 = Index Array(array=w720, index=0) -> (element=w713:dbl)
              n407 = local write "Z Axis Position (µm)"(w713) -> ()
              n408 = local write "Y Axis Position (µm)"(w712) -> ()
              n409 = local write "X Axis Position (µm)"(w711) -> ()
              n410 = Unbundle By Name(w745) -> ("XY Correction Active"=w735:bool, "XY Drift Threshold"=w762:dbl, "PID Values"=w760:dbl[])
              n411 = local read "Measured Y Position cc (px)"() -> (w756:dbl)
              n412 = local read "Measured X Position cc (px)"() -> (w757:dbl)
              n413 = Unbundle By Name(w745) -> ("Z Correction Active"=w736:bool, "Z Drift Threshold"=w738:dbl, "PID Values"=w744:dbl[])
              n414 = local read "Target X Position cc (px)"() -> (w755:dbl)
              n415 = local read "Target Y Position cc (px)"() -> (w754:dbl)
              n416 = Array To Cluster(array=w760) -> (cluster=w761:T21)
              n417 = local read "pixel size (µm)"() -> (w763:dbl)
              n418 = Array To Cluster(array=w744) -> (cluster=w743:T21)
              n419 = Build Array(w761) -> (w758:T22)
              n420 = Build Array(w755, w754) -> (w752:dbl[])
              n421 = Build Array(w757, w756) -> (w753:dbl[])
              n422 = local read "Measured Z (µm)"() -> (w740:dbl)
              n423 = local read "Target Z (µm)"() -> (w741:dbl)
              n424 = Divide(x=w762, y=w763) -> (x/y=w750:dbl)
              n425 = Subtract(x=w753, y=w752) -> (x-y=w751:dbl[])
              n426 = call-poly <vilib>:"PID.vi"("PID gains"=w758, "process variable"=w753, "setpoint"=w752) -> ("output"=→"dxy (px)":dbl[])  [unwired: 7 in, 1 out]
              n427 = Build Array(w750, w750) -> (w749:dbl[])
              n428 = Absolute Value(x=w751) -> (abs(x)=w748:dbl[])
              n429 = Subtract(x=w740, y=w741) -> (x-y=w742:dbl)
              n430 = call-poly <vilib>:"PID.vi"("PID gains"=w743, "process variable"=w740, "setpoint"=w741) -> ("dt out (s)"=→"dt z (s)":dbl, "output"=→"dz (µm)":dbl)  [unwired: 7 in]
              n431 = Greater?(x=w748, y=w749) -> (0:w747:bool[])
              n432 = Absolute Value(x=w742) -> (abs(x)=w739:dbl)
              n433 = Or Array Elements(Boolean array=w747) -> (logical OR=w746:bool)
              n434 = Greater?(x=w739, y=w738) -> (0:w737:bool)
              n435 = And(x=w735, y=w746) -> (x .and. y?=w730:bool)
              n436 = And(x=w736, y=w737) -> (x .and. y?=w729:bool)
              n437 = Build Array(w730, w729) -> (w731:bool[])
              n438 = Boolean Array To Number(Boolean array=w731) -> (number=w732:u32)
              n439 = case shown="2" w732 {
                tunnel: [4Pi_Obj_Lock_-_Actions."Update Plots" ("x") 4Pi_Obj_Lock_-_Actions."Move XY" ("x") 4Pi_Obj_Lock_-_Actions."Move Z" ("x") 4Pi_Obj_Lock_-_Actions."Move XYZ" ("x")] -> w728
                tunnel: [w764 TRUE FALSE w772] -> w726
                tunnel: [w764 FALSE TRUE w772] -> w725
                frame 0, Default {
                  w764 = FALSE
                  # "XYZ within limits, no move"
                }
                frame 1 {
                  # "X or Y outside limit, move XY"
                }
                frame 2 {
                  # "Sigma X / Y outside limit, move Z"
                }
                frame 3 {
                  w772 = TRUE
                  # "XYZ outside limit, move all"
                }
              }
              n440 = local write "XY Move"(w726) -> ()
              n441 = local write "Z Move"(w725) -> ()
            }
            frame "Move XYZ", "Move XY" {
              w806 = 2.0
              # "Initial XY stage positions"
              # "Check if move will go beyond ±2 µm of the original positions"
              n442 = case shown="True" TRUE {
                tunnel: w784 -> [_ w827]
                tunnel: [w825 w826] -> w779
                frame False {
                  n443 = local read "dxy (px)"() -> (w825:dbl[])
                }
                frame True {
                  # "Get XY Diff Values"
                  n444 = Array Subset(array=w827, index (row)=0 ("index"), length (row)=2 ("length"), index (col)=2 ("index")) -> (w828:dbl[][])  [unwired: 1 in]
                  n445 = Index Array(array=w828, index (col)=0 ("disabled index (col)")) -> (element=w826:dbl[])  [unwired: 1 in]
                }
              }
              n446 = Get Notifier Status(notifier=w823) -> (notifier out=w822:refnum<notifier>, current notification=w821:T8)  [unwired: 1 in, 3 out]
              n447 = Unbundle By Name(w821) -> ("Abort If Error"=w814:bool, "XY Stage Move Limit (µm)"=w817:dbl)
              n448 = Array Subset(array=w784, index (row)=0 ("index"), length (row)=2 ("length"), index (col)=3 ("index"), length (col)=1 ("length")) -> (w783:dbl[][])
              n449 = Index Array(array=w783, index (col)=0 ("disabled index (col)")) -> (element=w781:dbl[])  [unwired: 1 in]
              n450 = Equal?(x=4Pi_Obj_Lock_-_Actions."Move XYZ", y=w794) -> (x = y?=w792:bool)
              n451 = Build Array("X Update Scale Factor", "Y Update Scale Factor") -> (w775:dbl[])
              n452 = Select(t=4Pi_Obj_Lock_-_Actions."Move Z" ("x"), s=w792, f=4Pi_Obj_Lock_-_Actions."Update Plots") -> (s? t:f=w789:T6)
              n453 = Multiply(x=w779, y=w775) -> (x*y=w778:dbl[])
              n454 = call "Stages Messenger.vi"("Stage Notifier Name"=w798, "Actions"=Stage_Actions."Get Position") -> ("Stage Notifier Name (Dup)"=w797:string, "Positions"=w796:dbl[])  [unwired: 9 in, 3 out]
              n455 = call "4Pi Obj Lock - Rotate Flip XY.vi"("XY Amounts"=w778, "Flip XY"="Flip XY Axis", "Invert X"="Invert X Axis", "Invert Y"="Invert Y Axis") -> ("45° Rotated XY"=w780:dbl[])  [unwired: 11 in]
              n456 = Add(x=w796, y=w780) -> (x+y=w795:dbl[])
              n457 = Add(x=w781, y=w806) -> (x+y=w804:dbl[])
              n458 = Subtract(x=w781, y=w806) -> (x-y=w805:dbl[])
              n459 = Absolute Value(x=w780) -> (abs(x)=w816:dbl[])
              n460 = Greater?(x=w817, y=w816) -> (0:w815:bool[])
              n461 = In Range and Coerce(upper limit=w804, x=w795, lower limit=w805) -> (In Range?=w803:bool[])  [unwired: 1 out]
              n462 = And Array Elements(Boolean array=w815) -> (logical AND=w802:bool)
              n463 = And Array Elements(Boolean array=w803) -> (logical AND=w800:bool)
              n464 = And(x=w802, y=w800) -> (x .and. y?=w801:bool)
              n465 = Not(x=w801) -> (.not. x?=→"Move Limit Error":bool)
              n466 = case shown="True" w801 {
                tunnel: w780 -> [_ w843]
                tunnel: w814 -> [w837 _]
                tunnel: [w835 w840] -> w813
                tunnel: w797 -> [_ w842]
                tunnel: [dbl[] [-1.0, -1.0] ("Positions") w841] -> w811
                tunnel: w789 -> [w833 w840]
                frame False {
                  n467 = Select(t=4Pi_Obj_Lock_-_Actions."Abort" ("x"), s=w837, f=w833) -> (s? t:f=w835:T6)
                }
                frame True {
                  n468 = Wait (ms)(milliseconds to wait=u32 100) -> ()  [unwired: 1 out]
                  n469 = call "Stages Messenger.vi"("Stage Notifier Name"=w842, "Actions"=Stage_Actions."MVR", "Setpoint"=w843, "Axis"=bool[] [TRUE, TRUE], "Exit While Busy?"=FALSE) -> ("Positions"=w841:dbl[])  [unwired: 6 in, 4 out]
                }
              }
              n470 = Index Array(array=w811, index #1=0 ("index"), index #2=1 ("index")) -> (element #1=→"X Axis Position (µm)":dbl, element #2=→"Y Axis Position (µm)":dbl)
            }
            frame "Move Z" {
              w861 = 2.0 ("y")
              # "Initial Z stage position"
              n471 = Get Notifier Status(notifier=w879) -> (notifier out=w878:refnum<notifier>, current notification=w880:T8)  [unwired: 1 in, 3 out]
              n472 = case shown="True" TRUE {
                tunnel: [w882 w885] -> w873
                tunnel: w855 -> [_ w883]
                frame False {
                  n473 = local read "dz (µm)"() -> (w882:dbl)
                }
                frame True {
                  w884 = 0 ("disabled index (col)")
                  # "Get sx/sy Diff Value"
                  n474 = Array Subset(array=w883, index (row)=2 ("index"), length (row)=1 ("length"), index (col)=2 ("index"), length (col)=1 ("length")) -> (w887:dbl[][])
                  n475 = Index Array(array=w887, index (row)=w884, index (col)=w884) -> (element=w885:dbl)
                }
              }
              n476 = Index Array(array=w855, index (row)=2, index (col)=3 ("disabled index (col)")) -> (element=w852:dbl)
              n477 = Unbundle By Name(w880) -> ("Abort If Error"=w860:bool, "Z Stage Move Limit (µm)"=w865:dbl)
              n478 = Multiply(x=w873, y="Z Update Scale Factor") -> (x*y=w870:dbl)
              n479 = Add(x=w852, y=w861) -> (x+y=w867:dbl)
              n480 = Subtract(x=w852, y=w861) -> (x-y=w866:dbl)
              n481 = call "Stages Messenger.vi"("Stage Notifier Name"=w876, "Actions"=Stage_Actions."Get Position") -> ("Stage Notifier Name (Dup)"=w862:string, "Positions"=w874:dbl[])  [unwired: 9 in, 3 out]
              n482 = Negate(x=w870) -> (-x=w871:dbl)
              n483 = Select(t=w871, s="Invert Z Axis", f=w870) -> (s? t:f=w851:dbl)
              n484 = Index Array(array=w874, index=0) -> (element=w872:dbl)
              n485 = Absolute Value(x=w851) -> (abs(x)=w848:dbl)
              n486 = Add(x=w851, y=w872) -> (x+y=w868:dbl)
              n487 = Greater?(x=w865, y=w848) -> (0:w864:bool)
              n488 = Greater?(x=w848, y=0.002) -> (0:w846:bool)
              n489 = In Range and Coerce(upper limit=w867, x=w868, lower limit=w866) -> (In Range?=w863:bool)  [unwired: 1 out]
              n490 = And(x=w864, y=w863) -> (x .and. y?=w859:bool)
              n491 = Not(x=w859) -> (.not. x?=w858:bool)
              n492 = case shown="True" w859 {
                tunnel: w862 -> [_ w900]
                tunnel: w860 -> [w894 _]
                tunnel: w851 -> [_ w899]
                tunnel: [w893 4Pi_Obj_Lock_-_Actions."Update Plots" ("x")] -> w857
                tunnel: [-1.0 ("Position") w898] -> w856
                tunnel: w846 -> [_ w896]
                frame False {
                  n493 = Select(t=4Pi_Obj_Lock_-_Actions."Abort" ("x"), s=w894, f=4Pi_Obj_Lock_-_Actions."Update Plots") -> (s? t:f=w893:T6)
                }
                frame True {
                  n494 = case shown="True" w896 {
                    tunnel: w900 -> [w905 w910]
                    tunnel: w899 -> [_ w909]
                    tunnel: [w901 w907] -> w898
                    frame False {
                      n495 = call "Stages Messenger.vi"("Stage Notifier Name"=w905, "Actions"=Stage_Actions."Get Position") -> ("Positions"=w902:dbl[])  [unwired: 9 in, 4 out]
                      n496 = Index Array(array=w902, index=0) -> (element=w901:dbl)
                    }
                    frame True {
                      n497 = Build Array(w909) -> (w908:dbl[])
                      n498 = flat-sequence {
                        tunnel: w910 -> [w917]
                        tunnel: w908 -> [w916]
                        tunnel: [w912] -> w906
                        tunnel: [w920] -> w907
                        tunnel: w906 -> [w920]
                        frame #0 {
                          n499 = call "Stages Messenger.vi"("Stage Notifier Name"=w917, "Actions"=Stage_Actions."MVR", "Setpoint"=w916, "Axis"=bool[] [TRUE], "Exit While Busy?"=FALSE) -> ("Positions"=w914:dbl[])  [unwired: 6 in, 4 out]
                          n500 = Index Array(array=w914, index=0) -> (element=w912:dbl)
                        }
                        frame #1 {
                          n501 = Wait (ms)(milliseconds to wait=u32 150) -> ()  [unwired: 1 out]
                        }
                      }
                    }
                  }
                }
              }
              "Z Axis Position (µm)" <- w856
              n502 = local write "Move Limit Error"(w858) -> ()
            }
            frame "Update Plots" {
              (unwired) 0 ("index")
              # "Current Values"
              # "Target Values"
              n503 = Get Notifier Status(notifier=w1006) -> (notifier out=w1005:refnum<notifier>, current notification=w1007:T8)  [unwired: 1 in, 3 out]
              n504 = Unbundle By Name(w1007) -> ("Z Drift Threshold"=w998:dbl, "XY Drift Threshold"=w997:dbl)
              n505 = local read "X Axis Position (µm)"() -> (w992:dbl)
              n506 = local read "Y Axis Position (µm)"() -> (w991:dbl)
              n507 = local read "Z Axis Position (µm)"() -> (w990:dbl)
              n508 = Index Array(array=w987, index (col)=0 ("disabled index (col)")) -> (element=w984:dbl[])  [unwired: 1 in]
              n509 = Index Array(array=w987, index (col)=1 ("disabled index (col)")) -> (element=w985:dbl[])  [unwired: 1 in]
              n510 = Index Array(array=w987, index (col)=3 ("disabled index (col)")) -> (element=w988:dbl[])  [unwired: 1 in]
              n511 = Subtract(x=w985, y=w984) -> (x-y=w983:dbl[])
              n512 = local read "Measured Y Position cc (px)"() -> (w970:dbl)
              n513 = local read "Measured X Position cc (px)"() -> (w969:dbl)
              n514 = local read "Target X Position cc (px)"() -> (w971:dbl)
              n515 = local read "Target Y Position cc (px)"() -> (w972:dbl)
              n516 = Build Array(w992, w991, w990) -> (w989:dbl[])
              n517 = Index Array(array=w983, index #1=0 ("index"), index #2=1 ("index"), index #3=2 ("index")) -> (element #1=w968:dbl, element #2=w967:dbl, element #3=w925:dbl)
              n518 = Subtract(x=w989, y=w988) -> (x-y=w986:dbl[])
              n519 = Build Array(w968, w967) -> (w957:dbl[])
              n520 = Index Array(array=w986, index #1=0 ("index"), index #2=1 ("index"), index #3=2 ("index")) -> (element #1=w950:dbl, element #2=w949:dbl, element #3=w975:dbl)
              n521 = Build Array(w969, w970) -> (w973:dbl[])
              n522 = Build Array(w971, w972) -> (w974:dbl[])
              n523 = Build Array(w950, w949) -> (w943:dbl[])
              n524 = Subtract(x=w973, y=w974) -> (x-y=w966:dbl[])
              n525 = Square Root(x=2.0) -> (sqrt(x)=w945:dbl)
              n526 = Select(t=w957, s=FALSE, f=w966) -> (s? t:f=w964:dbl[])
              n527 = Divide(x=w943, y=w945) -> (x/y=w944:dbl[])
              n528 = Multiply(x="pixel size (µm)", y=w957) -> (x*y=w953:dbl[])
              n529 = Multiply(x="pixel size (µm)", y=w964) -> (x*y=w963:dbl[])
              n530 = Index Array(array=w944, index #1=0 ("index"), index #2=1 ("index")) -> (element #1=w942:dbl, element #2=w941:dbl)
              n531 = Index Array(array=w963, index #1=0 ("index"), index #2=1 ("index")) -> (element #1=w960:dbl, element #2=w959:dbl)
              n532 = Index Array(array=w953, index #1=0 ("index"), index #2=1 ("index")) -> (element #1=w952:dbl, element #2=w951:dbl)
              n533 = local read "Invert X Axis"() -> (w931:bool)
              n534 = Add(x=w942, y=w941) -> (x+y=w940:dbl)
              n535 = Subtract(x=w942, y=w941) -> (x-y=w934:dbl)
              n536 = Negate(x=w940) -> (-x=w935:dbl)
              n537 = local read "Invert Y Axis"() -> (w930:bool)
              n538 = Negate(x=w934) -> (-x=w938:dbl)
              n539 = Negate(x=w935) -> (-x=w939:dbl)
              n540 = local read "CC Max Value"() -> (w923:dbl)
              n541 = local read "Flip XY Axis"() -> (w932:bool)
              n542 = Select(t=w938, s=w930, f=w934) -> (s? t:f=w936:dbl)
              n543 = Select(t=w939, s=w931, f=w935) -> (s? t:f=w937:dbl)
              n544 = Bundle("CC Max Value"=w923) -> (→"CC Max":cluster{"CC Max Value":dbl})  [unwired: 1 in]
              n545 = Build Array(w937, w936) -> (w933:dbl[])
              n546 = case shown="True" w932 {
                tunnel: w933 -> [w1010 w1012]
                tunnel: [w1010 w1011] -> w928
                frame False {
                }
                frame True {
                  n547 = Reverse 1D Array(array=w1012) -> (reversed array=w1011:dbl[])
                }
              }
              n548 = Index Array(array=w928, index #2=1 ("index")) -> (element #1=w927:dbl, element #2=w926:dbl)  [unwired: 1 in]
              n549 = call "4Pi Obj Lock - 1 Values Organize Plot Data.vi"("Target 01"=0.0, "Value Limit"=w997, "Current 2"=w952, "Current 01"=w960, "Stage Pos"=w927) -> ("plot value"=→"X Target and Fit Position (µm)":T2)  [unwired: 10 in]
              n550 = Multiply(x=w925, y="Metric scale sx/sy") -> (x*y=w924:dbl)
              n551 = local read "Measured Z (µm)"() -> (w978:dbl)
              n552 = call "4Pi Obj Lock - 1 Values Organize Plot Data.vi"("Target 01"=0.0, "Value Limit"=w997, "Current 2"=w951, "Current 01"=w959, "Stage Pos"=w926) -> ("plot value"=→"Y Target and Fit Position (µm)":T2)  [unwired: 10 in]
              n553 = Select(t=w924, s=FALSE, f=w978) -> (s? t:f=w976:dbl)
              n554 = call "4Pi Obj Lock - 1 Values Organize Plot Data.vi"("Target 01"=0.0, "Value Limit"=w998, "Current 2"=w924, "Current 01"=w976, "Stage Pos"=w975) -> ("plot value"=→"Z Target and Fit Value (µm)":T2)  [unwired: 10 in]
            }
            frame "Delay" {
              n555 = Get Notifier Status(notifier=w1018) -> (notifier out=w1016:refnum<notifier>, current notification=w1019:T8)  [unwired: 1 in, 3 out]
              n556 = Unbundle By Name(w1019) -> ("Update Delay (ms)"=w1015:i32)
              n557 = while {
                tunnel: w1016 -> [w1031]
                tunnel: w1015 -> [w1028]
                tunnel: [w1024] -> w1014
                i -> [w1029]
                stop <- w1022 stop-if-true
                n558 = Get Notifier Status(notifier=w1031) -> (notifier out=w1024:refnum<notifier>, current notification=w1027:T8)  [unwired: 1 in, 3 out]
                n559 = Greater Or Equal?(x=w1029, y=w1028) -> (x >= y?=w1023:bool)
                n560 = Wait (ms)(milliseconds to wait=u32 1) -> ()  [unwired: 1 out]
                n561 = Unbundle By Name(w1027) -> ("Actions"=w1026:T6)
                n562 = Equal?(x=w1026, y=4Pi_Obj_Lock_-_Actions."Abort") -> (x = y?=w1021:bool)
                n563 = Or(x=w1021, y=w1023) -> (x .or. y?=w1022:bool)
              }
            }
            frame "Abort" {
              w1035 = 0.0 ("Target X Position (px)")
              n564 = Get Notifier Status(notifier=w1041) -> (notifier out=w1045:refnum<notifier>, current notification=w1044:T8)  [unwired: 1 in, 3 out]
              n565 = call "Camera Messenger.vi"("Notifier Name"=w1033, "General Camera Actions"=Generic_Camera_Actions."Abort") -> ()  [unwired: 8 in, 6 out]
              n566 = Bundle By Name(cluster=w1044, "Running?"=FALSE, "Actions"=4Pi_Obj_Lock_-_Actions."Exit Loop") -> (w1042:T8)
              n567 = Send Notification(notification=w1042, notifier=w1045) -> (notifier out=w1040:refnum<notifier>)  [unwired: 1 in, 1 out]
              n568 = local write "Start Lock"(FALSE ("Start Lock")) -> ()
              n569 = local write "Measured X Position (px)"(w1035) -> ()
              n570 = local write "Measured Y Position (px)"(w1035) -> ()
              n571 = local write "Target X Position (px)"(w1035) -> ()
              n572 = local write "Target Y Position (px)"(w1035) -> ()
              n573 = local write "Measured sx/sy"(w1035) -> ()
              n574 = local write "Target sx/sy"(w1035) -> ()
            }
            frame "Exit Loop" {
            }
            frame "Quit" {
              n575 = Get Notifier Status(notifier=w1051) -> (notifier out=w1050:refnum<notifier>, current notification=w1058:T8)  [unwired: 1 in, 3 out]
              n576 = Unbundle By Name(w1058) -> ("Ref Stack (SGL)"=w1057:T9[], "Cur Image (SGL)"=w1056:T9, "Tmp Image FFT (CSG)"=w1055:T9[], "CC Image (SGL)"=w1054:T9, "Ref FFT Stack (CSG)"=w1052:T9[])
              n577 = Release Notifier(notifier=w1050, force destroy? (F)=TRUE) -> ()  [unwired: 1 in, 3 out]
              n578 = Build Array (concatenate)(w1057, w1056, w1055, w1054, w1052) -> (w1053:T9[])
              n579 = for {
                tunnel: w1053 -> [w1063] mode=indexing
                n580 = call "IMAQ Dispose"("Image"=w1063) -> ()  [unwired: 5 in, 1 out]
              }
            }
          }
          n581 = Get Notifier Status(notifier=w235) -> (current notification=w234:T8, error out=w229:errorcluster)  [unwired: 1 in, 3 out]
          n582 = Unbundle By Name(w234) -> ("Actions"=w233:T6)
          n583 = Unbundle By Name(w229) -> ("status"=w227:bool)
          n584 = Equal?(x=w232, y=w233) -> (x = y?=w228:bool)
          n585 = Or(x=w228, y=w227) -> (x .or. y?=w226:bool)
          n586 = Select(t=w232, s=w226, f=w231) -> (s? t:f=w230:T6)
        }
      }
      n587 = local write "Quit"(w209) -> ()
    }
    frame Error {
    }
  }
  n588 = control-ref of="This VI"() -> (w87:refnum<vi>)
  n589 = property class="VI"(reference=w87) -> (reference out=w96:refnum<vi>, "Panel"=w88:refnum<vi>)  [unwired: 1 in, 1 out]
  n590 = property class="Pnl"(reference=w88) -> ("Decos[]"=w86:refnum<vi>[], "Panes[]"=w92:refnum<vi>[])  [unwired: 1 in, 2 out]
  n591 = Array Size(array=w86) -> (size(s)=w84:i32)
  n592 = Decrement(x=w84) -> (x-1=w85:i32)
  n593 = Index Array(array=w92, index=0) -> (element=w91:refnum<vi>)
  n594 = Index Array(array=w86, index=w85) -> (element=w94:refnum<vi>)
  n595 = property class="VI"(reference=w96) -> (reference out=w98:refnum<vi>, "Front Panel.PanelBounds"=w99:T23)  [unwired: 1 in, 1 out]
  n596 = property class="Decor"(reference=w94) -> ("Bounds"=w97:T24)  [unwired: 1 in, 2 out]
  n597 = property class="Pane"(reference=w91, "Origin"=T11 {"Horizontal"=0, "Vertical"=0}, "HorizScrollbarVisibility"=w95, "VertScrollbarVisibility"=w95) -> ()  [unwired: 1 in, 2 out]
  n598 = Unbundle By Name(w97) -> ("Width"=w102:u32, "Height"=w105:u32)
  n599 = control-ref of="Quit"() -> (w89:refnum<vi>)
  n600 = To Word Integer(number=w102) -> (16bit integer=w104:i16)
  n601 = To Word Integer(number=w105) -> ()  [unwired: 1 out]
  n602 = property class="Bool (strict)"(reference=w89) -> ("Height"=w107:u32, "Top"=w108:i32)  [unwired: 1 in, 2 out]
  n603 = Unbundle By Name(w99) -> ("Left"=w101:i16, "Top"=w112:i16)
  n604 = To Word Integer(number=w107) -> (16bit integer=w110:i16)
  n605 = To Word Integer(number=w108) -> (16bit integer=w111:i16)
  n606 = Add(x=w101, y=w104) -> (x+y=w103:i16)
  n607 = Compound Arithmetic op=ADD(w112, w110, w111, i16 12 ("y")) -> (w106:i16)
  n608 = Bundle By Name(cluster=w99, "Right"=w103, "Bottom"=w106) -> (w100:T23)
  n609 = property class="VI"(reference=w98, "Front Panel.PanelBounds"=w100) -> ()  [unwired: 1 in, 2 out]
